vi "Process.vi"(8 "error in":errorcluster, 11 "Instrument.DAQ":refnum<class "Instrument.DAQ.lvclass">) -> (0 "error out":errorcluster, 3 "Instrument.DAQ out":refnum<class "Instrument.DAQ.lvclass">)   [LabVIEW 2019, in "Instrument.Lockin.lvlib" / "Instrument.DAQ.lvclass"]
doc: "---------------------------------------------------------------\nJKI State Machine Objects™\nhttp://jki.net/state-machine-objects/\nCopyright (C) 2005-2015, JKI <info@jki.net>\nALL RIGHTS RESERVED"
uses:
  Instrument.DAQ.lvclass
  C:/Program Files/National Instruments/LabVIEW 2019/vi.lib/JKI/JKI SMO/SMO/SMO.lvclass
  Typedefs/Status--enum.ctl
  Typedefs/DAQ.Config.AO.Range--enum.ctl
  Typedefs/DAQ.Type--enum.ctl
  Typedefs/DAQ.Config.AI.Coupling--enum.ctl
  Typedefs/DAQ.Config.AI.Range--enum.ctl
  DAQmx/typedefs/DAQmx.Status--enum.ctl
  Instrument.DAQ.lvclass/Instrument.DAQ.ctl
  Typedefs/Channel.Gain--Cluster.ctl
  Generator/typedefs/Generator.Sweep Status--enum.ctl
  Typedefs/PublicEvents--DAQ.getSweepWaveforms.ctl
  Typedefs/Results--Cluster.ctl
  <vilib>/JKI/JKI SMO/SMO/SMO.lvclass/SMO.ctl
  Typedefs/PrivateEvents--DAQ.setCalibration.ctl
  support/Simulate/Waveguide Model--Cluster.ctl
  Typedefs/PublicEvents--DAQ.getWaveforms.ctl
  Generator/typedefs/Generator.Command--enum.ctl
  6518129d-eb05-4862-8e0f-948d46b99fe2.vi
  19e91f76-1afa-420f-8f76-37c2ee2699b4.vi
  <vilib>/JKI/JKI SMO/SMO/Private/ReftoDVR--SMO.vi
  <vilib>/dlg_ctls.llb/Space Constant.vi
  <vilib>/AdvancedString/1D String Array to Delimited String.vi
  <vilib>/measure/madcrms.llb/Basic Averaged DC-RMS for N Chan.vi
  <vilib>/JKI/JKI SMO/SMO/SMO.lvclass
  <vilib>/measure/NI_MAPro.lvlib
  Instrument.Lockin/Instrument.Lockin.lvclass
  <userlib>/LevyLab/Debug/Debug.lvlib
  DAQmx/DAQmx.lvclass
  DSP/DSP.lvclass
  Waveform.Attributes/Waveform.Attributes.lvlib
  Generator/Generator.lvclass
panel:
  in  "Tab Control":enum32{"Default", "Advanced"}(tab)
  out "Sweep Chart":dbl(graph)
  out "Generator Chart":u32(graph)
  out "DSP Chart":dbl(graph)
  out "Total Chart":dbl(graph)
  out "sweep status":string
  out "Sweep Start":dbl format="%<%.3X>T"
  out "Status":T1=enum."created"
  in  "Calibrate Phase":bool
  in  "Reset Phase":bool
  out "Total (s)":dbl format="%06_6p"
  in  "Auto Phase":bool
  in  "Zero Offset":bool
  in  "Measure Offset":bool
  out "s.h.":string caption="State History"
  out "Payload":variant
  out "Generate (ms)":u32
  out "DSP (s)":dbl format="%0#6_6p"
  in  "Reset REF":bool
  out "Method":string
  out "DAQmx Status":T2
  out "start sweep":string
  out "reset":string
  in  "DAQ AO":T5(array[cluster]) {"configuration" items=["Default"=-1, "Differential"=10106, "Pseudodifferential"=12529]}
  in  "DAQ AI":T8(array[cluster]) {"configuration" items=["default"=-1, "Differential"=10106, "Pseudodifferential"=12529]; "Coupling" items=[""=0, "AC"=10045, "DC"=10050, "GND"=10066]}
  # "For instructions on how to use the JKI State Machine Objects, examples and video tutorials, visit:\nhttp://jki.net/state-machine-objects/\n\nJKI State Machine Objects™\nhttp://jki.net/state-machine-objects/\nCopyright (C) 2005-2015, JKI <info@jki.net>\nALL RIGHTS RESERVED"
  # "DAQ"
  # "State"
  # "Messages"
  # "Sweep"
  # "Controls"
  # "Timing"
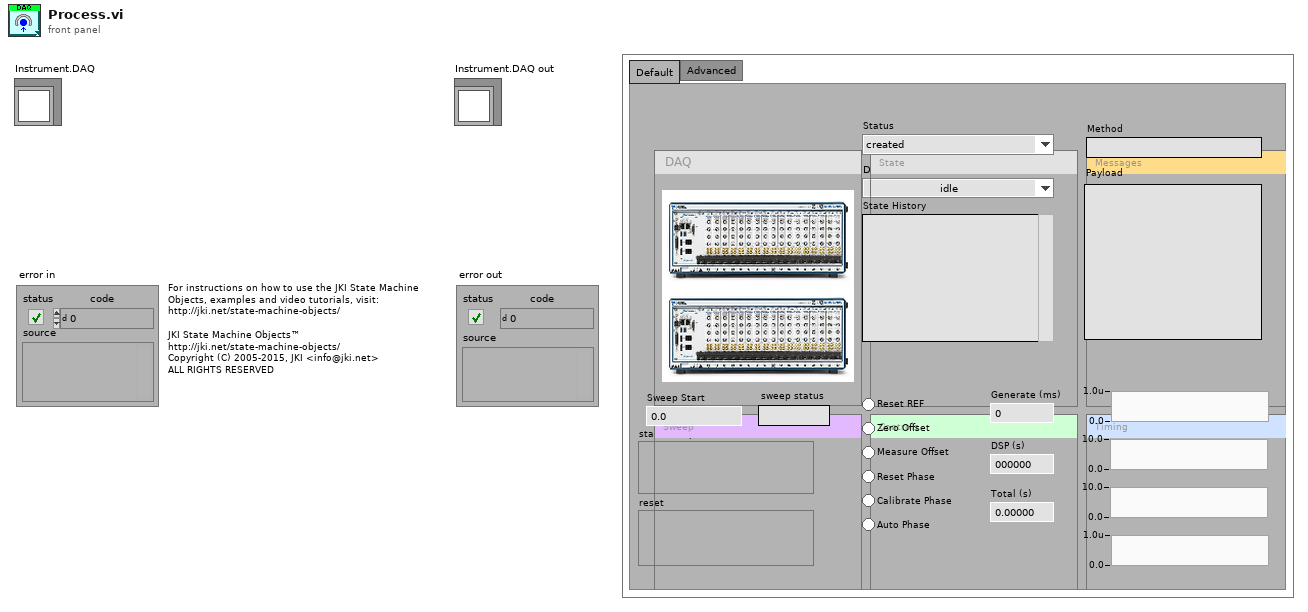
[diagram p1: front panel]
types:
  T1 = typedef "Instrument.Lockin.lvlib/Instrument.DAQ.lvclass/Status--enum.ctl" = enum16{"idle", "created", "started", "stopped", "sweeping"}
  T2 = typedef "DAQmx.lvclass/DAQmx.Status--enum.ctl" = enum16{"idle", "calibrating", "configuring", "creating", "created", "starting", "started", "stopping", "stopped", "clearing", "error"}
  T3 = typedef "Instrument.Lockin.lvlib/Instrument.DAQ.lvclass/DAQ.Config.AO.Range--enum.ctl" = enum16{"±0.1", "±1.0", "±3.5", "±10.0", ""}
  T4 = typedef "Instrument.Lockin.lvlib/Instrument.DAQ.lvclass/DAQ.Type--enum.ctl" = enum16{"None", "USB-4431", "PXI-446x"}
  T5 = cluster{"Channel":tag, "Range":T3, "configuration":i32, "Type":T4}[]
  T6 = typedef "Instrument.Lockin.lvlib/Instrument.DAQ.lvclass/DAQ.Config.AI.Coupling--enum.ctl" = u16
  T7 = typedef "Instrument.Lockin.lvlib/Instrument.DAQ.lvclass/DAQ.Config.AI.Range--enum.ctl" = enum16{"±0.316", "±1.00", "±3.16", "±10.0", "±31.6", "±42.4", ""}
  T8 = cluster{"Channel":tag, "Coupling":T6, "Range":T7, "configuration":i32, "Type":T4}[]
  T9 = typedef "Instrument.Lockin.lvlib/Instrument.DAQ.lvclass/Channel.Gain--Cluster.ctl" = cluster{"Channel":string, "Gain":dbl}
  T10 = enum32{"invalid app kind", "Development System", "Run Time System", "Student Edition", "Embedded LabVIEW", "Evaluation", "Custom"}
  T11 = typedef "Instrument.Lockin.lvlib/Instrument.DAQ.lvclass/PublicEvents--DAQ.getSweepWaveforms.ctl" = cluster{"AO":waveform(dbl)[], "AI":waveform(dbl)[], "X":waveform(dbl)[], "Y":waveform(dbl)[]}
  T12 = enum32{"Invalid", "Standard", "Closed", "Hidden", "Minimized", "Maximized"}
  T13 = typedef "Generator.lvclass/Generator.Sweep Status--enum.ctl" = enum16{"idle", "initializing", "waiting", "sweeping", "stopping"}
  T14 = typedef "Instrument.Lockin.lvlib/Instrument.DAQ.lvclass/PrivateEvents--DAQ.setCalibration.ctl" = enum16{"Check", "Calibrate"}
  T15 = typedef "Instrument.Lockin.lvlib/Instrument.DAQ.lvclass/Waveguide Model--Cluster.ctl" = cluster{"I+":i32, "I-":i32, "V+":i32, "V-":i32, "Vsg":i32}
  T16 = typedef "Instrument.Lockin.lvlib/Instrument.DAQ.lvclass/PublicEvents--DAQ.getWaveforms.ctl" = cluster{"AO":waveform(dbl)[], "AI":waveform(dbl)[], "REF_X":waveform(dbl)[], "REF_Y":waveform(dbl)[], "X":waveform(dbl)[], "Y":waveform(dbl)[]}
  T17 = typedef "Generator.lvclass/Generator.Command--enum.ctl" = enum16{"start", "stop", "start sweep", "stop sweep"}
  T18 = typedef "Instrument.Lockin.lvlib/Instrument.DAQ.lvclass/Results--Cluster.ctl" = cluster{"Time Stamp":timestamp, "Results (Dictionary)":cluster{"key":string, "value":dbl[]}[]}
  T19 = cluster{"Core":cluster{"Current VI Reference":refnum<vi>, "Close Panel on Exit?":bool, "Last Error":cluster{"error":errorcluster, "previous state":string, "remaining states":string}, "Shutdown?":bool}, "SMO":refnum<class "Instrument.DAQ.lvclass">, "DAQ Status":T1, "DAQmx Status":T2, "Sweep Status":T13, "Results":T18, "SweepWaveforms":T11, "Measure Offset":bool, "Saved Amplitudes":dbl[]}
  T20 = typedef "Instrument.Lockin.lvlib/Instrument.DAQ.lvclass/DAQ.Config.AO--Cluster--Array.ctl" = cluster{"Channels":tag, "Range":T3, "terminal configuration":T21, "Type":T4}[]
  T21 = typedef "Instrument.Lockin.lvlib/Instrument.DAQ.lvclass/DAQ.TerminalConfiguration--ring.ctl" = i32
  T22 = cluster{"Channels":tag, "Range":T3, "terminal configuration":T21, "Type":T4}
  T23 = typedef "Instrument.Lockin.lvlib/Instrument.DAQ.lvclass/DAQ.Config.AI--Cluster--Array.ctl" = cluster{"Channels":tag, "Coupling":T6, "Range":T7, "terminal configuration":T21, "Type":T4}[]
  T24 = typedef "Instrument.Lockin.lvlib/Instrument.DAQ.lvclass/Simulation Mode--enum.ctl" = enum16{"AI = HW simulated", "AI = noise*AO", "AI = waveguide"}
  T25 = cluster{"AI Configuration":T23, "Simulation mode":T24}
  T26 = cluster{"Channels":tag, "Coupling":T6, "Range":T7, "terminal configuration":T21, "Type":T4}
  T27 = typedef "Instrument.Lockin.lvlib/Instrument.DAQ.lvclass/AO.Channel--Cluster--Array.ctl" = T28[]
  T28 = typedef "Instrument.Lockin.lvlib/Instrument.DAQ.lvclass/AO.Channel--Cluster.ctl" = cluster{"Enable?":bool, "Channel":i32, "Amplitude":dbl, "Offset":dbl, "Frequency":dbl, "Phase":dbl, "Function":T29, "Sweeping?":bool, "Limit AC":bool, "Limit DC?":bool, "Duty Cycle":bool}
  T29 = typedef "Instrument.Lockin.lvlib/Instrument.DAQ.lvclass/AO.Channel.Function--Enum.ctl" = enum16{"sine", "square", "triangle", "saw"}
  T30 = typedef "Instrument.Lockin.lvlib/Instrument.DAQ.lvclass/AI.Channel--Cluster--Array.ctl" = T31[]
  T31 = typedef "Instrument.Lockin.lvlib/Instrument.DAQ.lvclass/AI.Channel--Cluster.ctl" = cluster{"Enable?":bool, "Channel":i32, "References":u16[], "reference index":i32}
  T32 = typedef "Instrument.Lockin.lvlib/Instrument.DAQ.lvclass/REF.Channel--Cluster--Array.ctl" = T33[]
  T33 = typedef "Instrument.Lockin.lvlib/Instrument.DAQ.lvclass/REF.Channel--Cluster.ctl" = cluster{"Enable?":bool, "Channel":i32, "Frequency":dbl, "Phase":dbl, "TC":dbl, "Roll-Off":i32}
  T34 = typedef "Instrument.Lockin.lvlib/Instrument.DAQ.lvclass/DAQ.Sampling--Cluster.ctl" = cluster{"Sampling":T35, "sample mode":i32, "Fs Mode":T36, "Fs Multiplier":dbl, "Refresh Rate (Hz)":dbl, "Decimation.PreDSP":i32, "Decimation.PostDSP":i32, "Fs.Output":dbl}
  T35 = typedef "Instrument.Lockin.lvlib/Instrument.DAQ.lvclass/DAQ.Sampling.Sampling--Cluster.ctl" = cluster{"Fs":dbl, "#s":i32}
  T36 = typedef "Instrument.Lockin.lvlib/Instrument.DAQ.lvclass/DAQ.Sampling.Fs Mode--enum.ctl" = enum16{"Manual", "Auto Fs", "Max Fs"}
  T37 = typedef "Instrument.Lockin.lvlib/Instrument.DAQ.lvclass/Sweep.Configuration--Cluster.ctl" = cluster{"sweepTime":dbl, "initialWaitTime":dbl, "returnToStart":bool, "sweepChannels":T38}
  T38 = typedef "Instrument.Lockin.lvlib/Instrument.DAQ.lvclass/Sweep.Channel--Cluster--Array.ctl" = T39[]
  T39 = typedef "Instrument.Lockin.lvlib/Instrument.DAQ.lvclass/Sweep.Channel--Cluster.ctl" = cluster{"Enable?":bool, "Channel":u16, "Start":dbl, "End":dbl, "Pattern":T40, "Table":dbl[]}
  T40 = typedef "Instrument.Lockin.lvlib/Instrument.DAQ.lvclass/Sweep.Pattern--Enum.ctl" = enum16{"Ramp /", "Ramp /\\", "Smooth Ramp _/", "Smooth Ramp _/\\_", "Table"}
  T41 = typedef "Instrument.Lockin.lvlib/Instrument.DAQ.lvclass/PrivateEvents--DAQ.measureOffset.ctl" = bool
  T42 = typedef "Instrument.Lockin.lvlib/Instrument.DAQ.lvclass/PrivateEvents--DAQ.zeroPhase.ctl" = bool
  T43 = typedef "Instrument.Lockin.lvlib/Instrument.DAQ.lvclass/Configuration.Prefilter--Cluster.ctl" = cluster{"60 Hz":bool, "Low Pass":bool, "Low Pass Cutoff (Hz)":dbl}
  T44 = typedef "Instrument.Lockin.lvlib/Instrument.DAQ.lvclass/Configuration.AmplitudeLimit--Cluster.ctl" = cluster{"Limit?":bool, "Limit (V)":dbl}
  T45 = typedef "Instrument.Lockin.lvlib/Instrument.DAQ.lvclass/Configuration.DCLimit--Cluster.ctl" = cluster{"Limit?":bool, "Limit (V)":dbl}
  T46 = typedef "Instrument.Lockin.lvlib/Instrument.DAQ.lvclass/Configuration.DutyCycle--Cluster.ctl" = cluster{"Option?":bool, "Duty Cycle (%)":dbl}
  T47 = typedef "Instrument.Lockin.lvlib/Instrument.DAQ.lvclass/Configuration.LinkFrequencies--Cluster.ctl" = cluster{"Link?":bool, "Frequency (Hz)":dbl}
  T48 = typedef "Instrument.Lockin.lvlib/Instrument.DAQ.lvclass/State--enum.ctl" = enum16{"start", "stop", "reset", "start sweep", "stop sweep"}
  T49 = typedef "Instrument.Lockin.lvlib/Instrument.DAQ.lvclass/PrivateEvents--DAQ.showUI.ctl" = bool
  T50 = typedef "DAQmx.lvclass/DeviceInfo--Cluster.ctl" = cluster{"DeviceName":string, "DevIsSimulated":bool, "DeviceSerialNumber":string, "ProductType":string, "ProductCategory":i32, "ProductNumber":u32, "ChassisNumber":u32, "SlotNumber":u32, "ChassisName":string, "ChassisSerialNumber":string, "DevTemp":dbl, "SelfCal.LastDate/Time":string, "SelfCal.LastTemp":dbl, "calibration due?":bool}
  T51 = cluster{"Active Device":string, "SelfCal.LastDate/Time":string, "SelfCal.LastTemp":dbl, "DevTemp":dbl, "calibration due?":bool}[]
  T52 = typedef "Instrument.Lockin.lvlib/Instrument.DAQ.lvclass/DAQ.Calibration--Cluster.ctl" = cluster{"Active Device":string, "SelfCal.LastDate/Time":dbl, "SelfCal.LastTemp":dbl, "DevTemp":dbl, "calibration due?":bool}
  T53 = typedef "eventsource.ctl" = u32
  T54 = typedef "DAQmx.lvclass/DAQ.Config.Timing.Sampling--Cluster.ctl" = cluster{"Fs":dbl, "#s":i32}
  T55 = typedef "DAQmx.lvclass/DAQ.Config.Timing.Fs Mode--enum.ctl" = enum16{"Manual", "Auto Fs", "Max Fs"}
  T56 = typedef "DAQmx.lvclass/DAQ.Config.AO--Cluster--Array.ctl" = T57[]
  T57 = typedef "DAQmx.lvclass/DAQ.Config.AO--Cluster.ctl" = cluster{"Channels":tag, "Range":T58, "output terminal configuration":i32, "Type":T59}
  T58 = typedef "DAQmx.lvclass/DAQ.Config.AO.Range--enum.ctl" = enum16{"±0.1", "±1.0", "±3.5", "±10.0", ""}
  T59 = typedef "DAQmx.lvclass/DAQ.Config.Device Type--enum.ctl" = enum16{"None", "USB-4431", "PXI-446x"}
  T60 = typedef "DAQmx.lvclass/DAQ.Config.AI--Cluster--Array.ctl" = T61[]
  T61 = typedef "DAQmx.lvclass/DAQ.Config.AI--Cluster.ctl" = cluster{"Channels":tag, "Coupling":T62, "Range":T63, "input terminal configuration":i32, "Type":T59}
  T62 = typedef "DAQmx.lvclass/DAQ.Config.AI.Coupling--enum.ctl" = u16
  T63 = typedef "DAQmx.lvclass/DAQ.Config.AI.Range--enum.ctl" = enum16{"±0.316", "±1.00", "±3.16", "±10.0", "±31.6", "±42.4", ""}
  T64 = typedef "Generator.lvclass/AO.Channel--Cluster--Array.ctl" = T65[]
  T65 = typedef "Generator.lvclass/AO.Channel--Cluster.ctl" = cluster{"Enable?":bool, "Channel":i32, "Amplitude":dbl, "Offset":dbl, "Frequency":dbl, "Phase":dbl, "Function":T66, "Sweeping?":bool, "Limit AC?":bool, "Limit DC?":bool, "Duty Cycle?":bool, "Duty Cycle":dbl}
  T66 = typedef "Generator.lvclass/AO.Channel.Function--Enum.ctl" = enum16{"sine", "square", "triangle", "saw"}
  T67 = cluster{"Current VI Reference":refnum<vi>, "Close Panel on Exit?":bool, "Last Error":cluster{"error":errorcluster, "previous state":string, "remaining states":string}, "Shutdown?":bool}
  T68 = typedef "Instrument.Lockin.lvlib/Instrument.DAQ.lvclass/DeviceInfo--Cluster.ctl" = cluster{"DeviceName":string, "DevIsSimulated":bool, "DeviceSerialNumber":string, "ProductType":string, "ProductCategory":i32, "ProductNumber":u32, "ChassisNumber":u32, "SlotNumber":u32, "ChassisName":string, "ChassisSerialNumber":string, "DevTemp":dbl, "SelfCal.LastDate/Time":string, "SelfCal.LastTemp":dbl, "calibration due?":bool}
  T69 = typedef "Instrument.Lockin.lvlib/Instrument.DAQ.lvclass/DAQ.Calibration--Cluster--Array.ctl" = T52[]
  T70 = typedef "Instrument.Lockin.lvlib/Instrument.DAQ.lvclass/DAQ.Configuration--Cluster--Array.ctl" = T71[]
  T71 = typedef "Instrument.Lockin.lvlib/Instrument.DAQ.lvclass/DAQ.Configuration--Cluster.ctl" = cluster{"Device":string, "Lockin.AO":string, "AO.Ch":string, "AO.Range":T3, "AO terminal config":T21, "Lockin.AI":string, "AI.Ch":string, "AI.Range":T7, "AI.Coupling":T6, "AI terminal config":T21}
  T72 = typedef "Instrument.Lockin.lvlib/Instrument.DAQ.lvclass/Channel.Gain--Cluster--Array.ctl" = T9[]
  T73 = typedef "Debug.lvlib/Attribute.Debug.lvclass/DebugBehavior.ctl" = enum16{"Normal", "Debug"}
  T74 = typedef "SMO.lvclass/Protected Events.ctl" = cluster{"StopProcesses":refnum<user-event>, "AbortProcesses":refnum<user-event>, "Config Changed":refnum<user-event>, "Dependency":refnum<user-event>}
  T75 = typedef "Instrument.Lockin.lvlib/Instrument.DAQ.lvclass/PrivateEvents--Cluster.ctl" = cluster{"setAOconfig":refnum<user-event>, "setAIconfig":refnum<user-event>, "setAO":refnum<user-event>, "setREF":refnum<user-event>, "setSampling":refnum<user-event>, "setState":refnum<user-event>, "setInputGain":refnum<user-event>, "setOutputGain":refnum<user-event>, "setSweep":refnum<user-event>, "measureOffset":refnum<user-event>, "zeroOffset":refnum<user-event>, "setPreFilter":refnum<user-event>, "autoConfigureDAQ":refnum<user-event>, "setCalibration":refnum<user-event>, "setAI":refnum<user-event>, "zeroPhase":refnum<user-event>, "setAmplitudeLimit":refnum<user-event>, "setLinkFrequencies":refnum<user-event>, "showUI":refnum<user-event>, "setInputOffset":refnum<user-event>, "setDCLimit":refnum<user-event>, "setDutyCycle":refnum<user-event>}
  T76 = typedef "DAQmx.lvclass/PublicEvents--Cluster.ctl" = cluster{"Status":refnum<user-event>, "Devices":refnum<user-event>, "Calibration":refnum<user-event>, "Timing":refnum<user-event>, "AOconfig":refnum<user-event>, "AIconfig":refnum<user-event>, "Waveforms":refnum<user-event>}
  T77 = typedef "Generator.lvclass/PublicEvents--Cluster.ctl" = cluster{"Status":refnum<user-event>, "SweepStatus":refnum<user-event>, "AOChannels":refnum<user-event>, "Waveforms":refnum<user-event>}
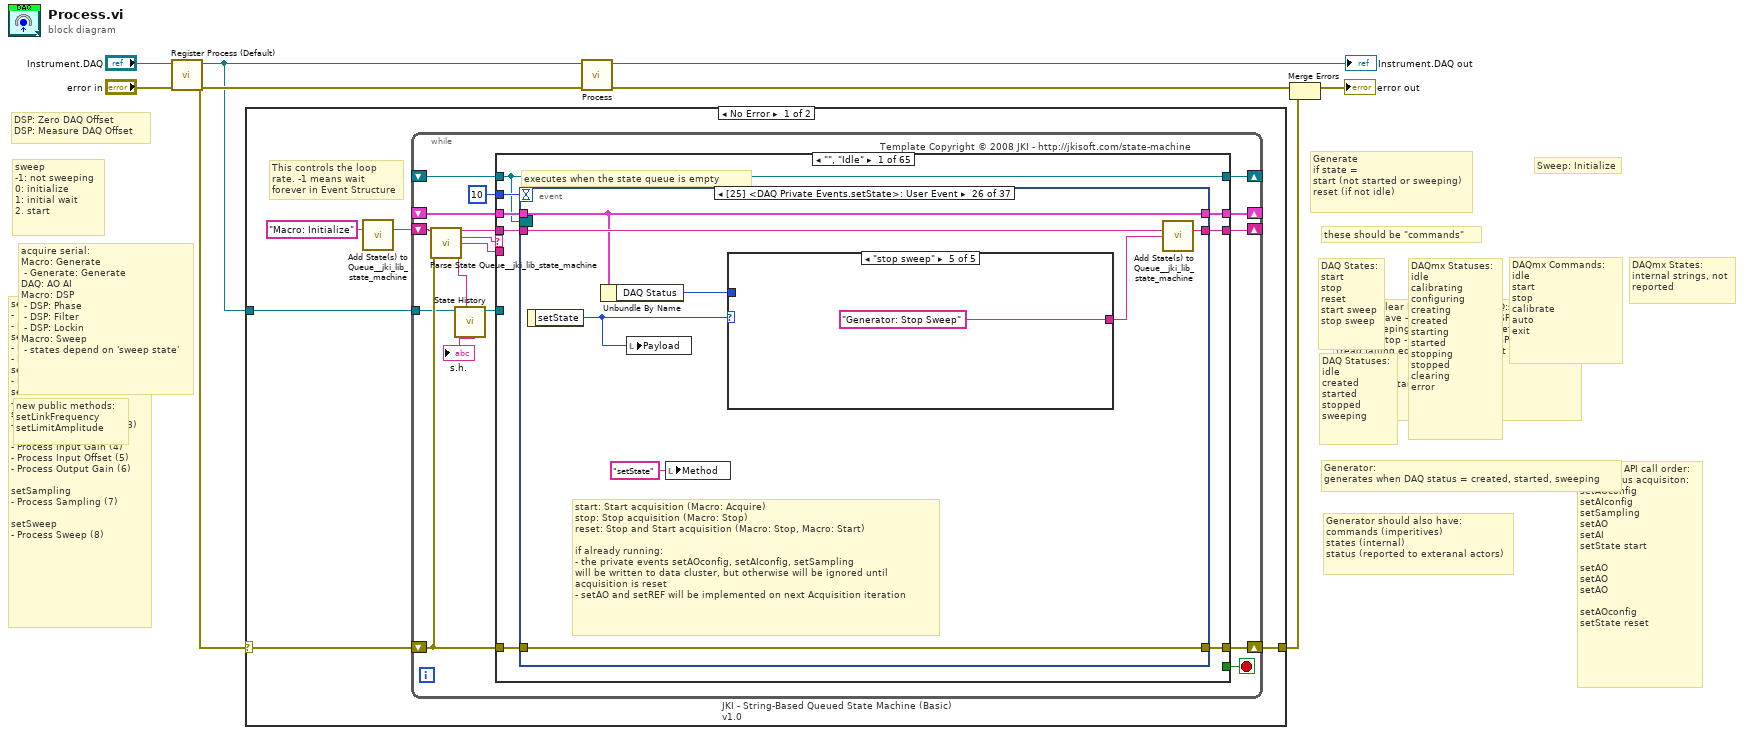
[diagram p0: block diagram]
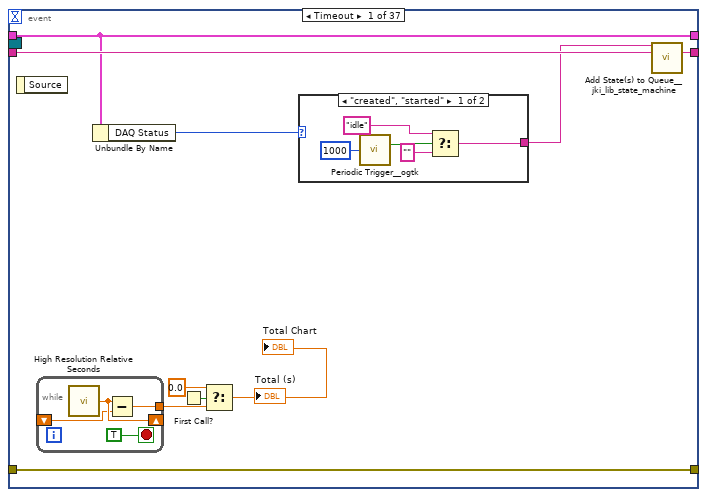
[diagram p2: hidden frame]
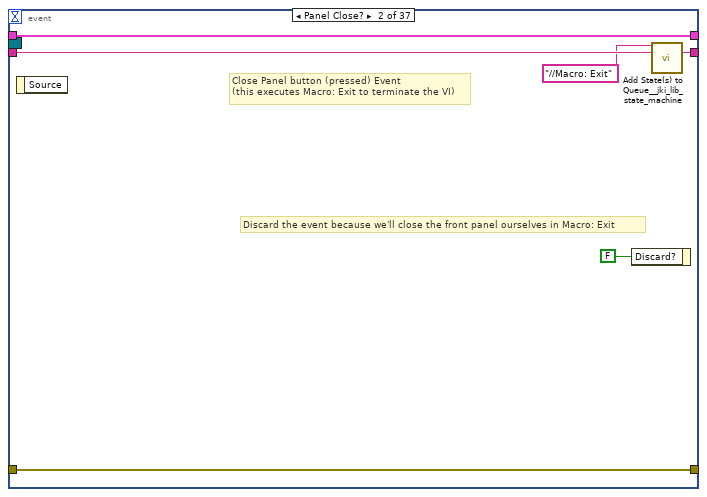
[diagram p4: hidden frame]
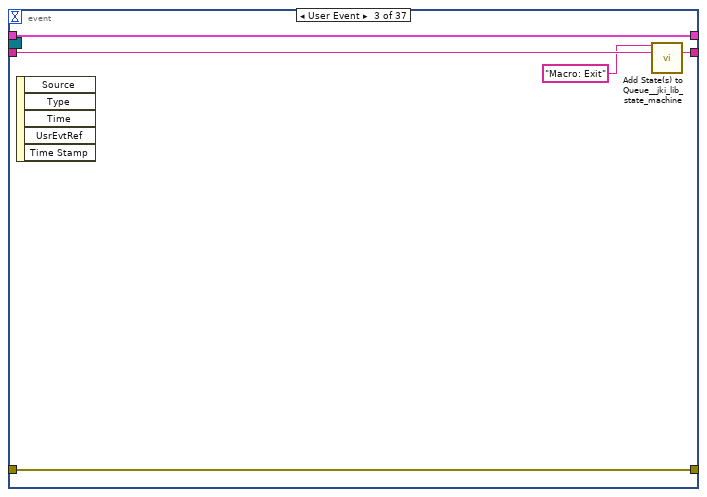
[diagram p5: hidden frame]
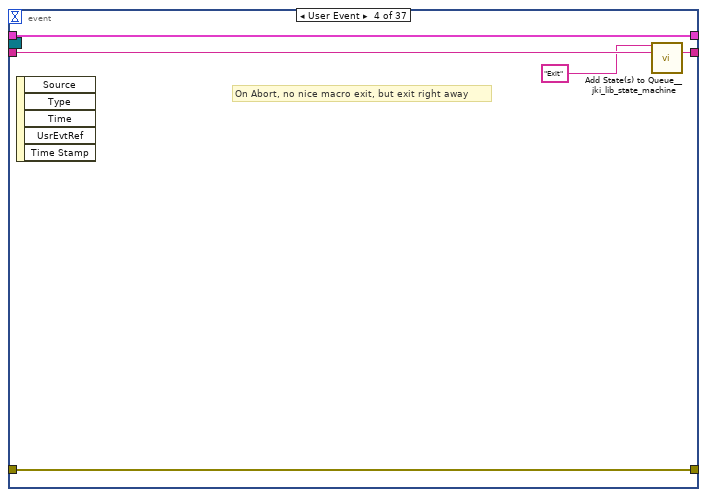
[diagram p6: hidden frame]
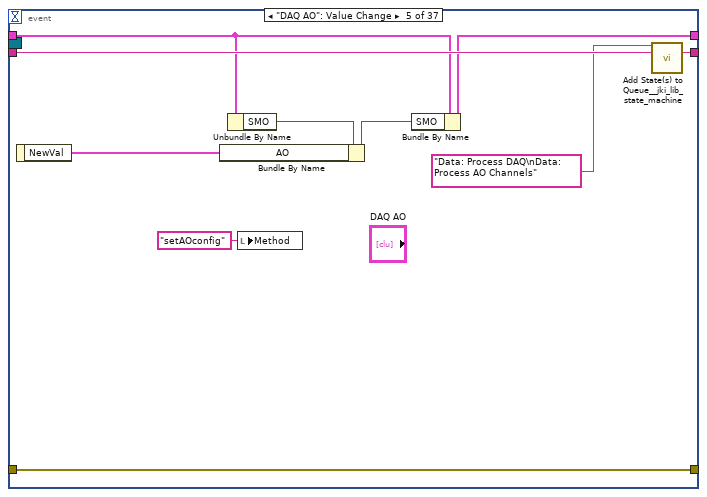
[diagram p7: hidden frame]
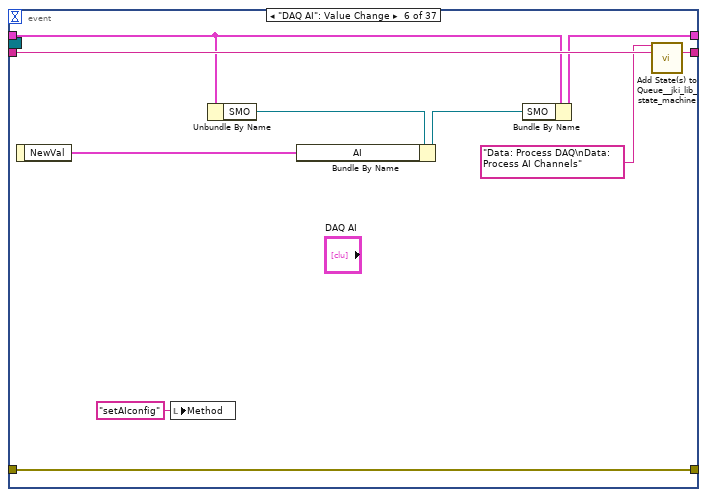
[diagram p8: hidden frame]
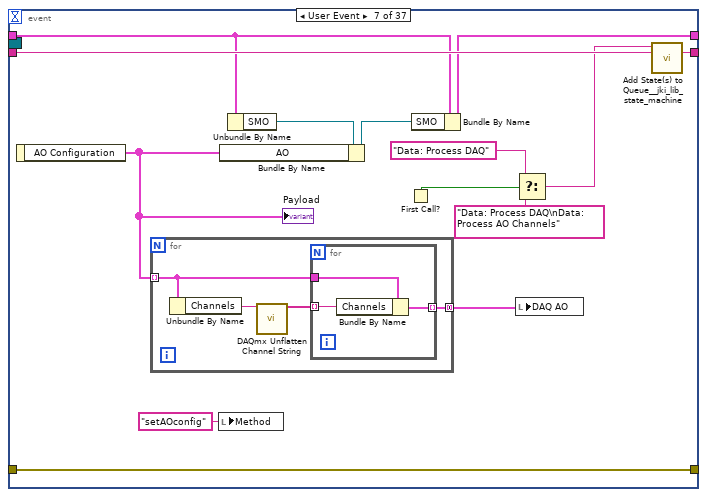
[diagram p9: hidden frame]
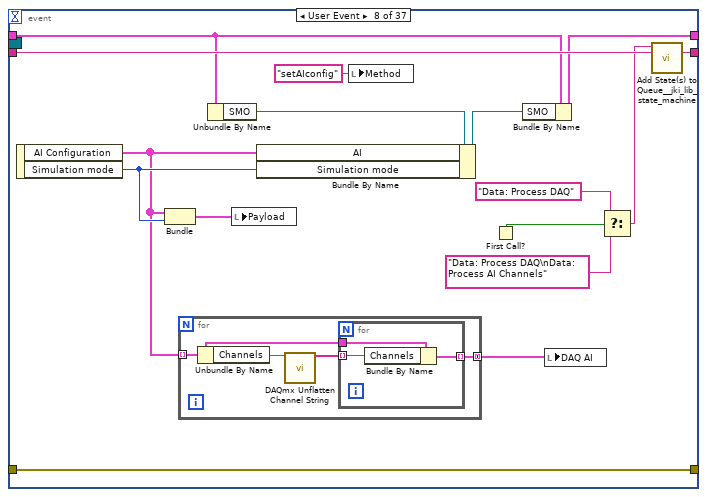
[diagram p10: hidden frame]
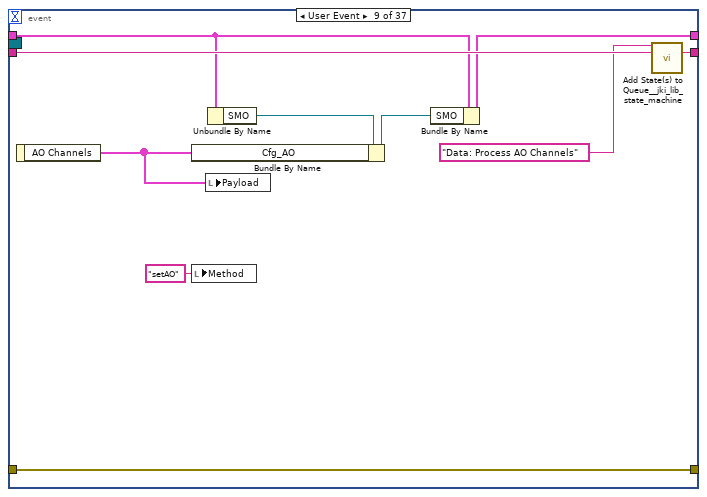
[diagram p11: hidden frame]
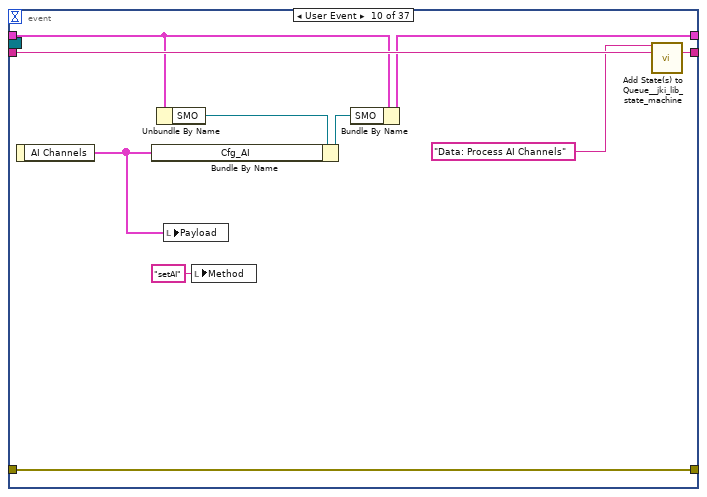
[diagram p12: hidden frame]
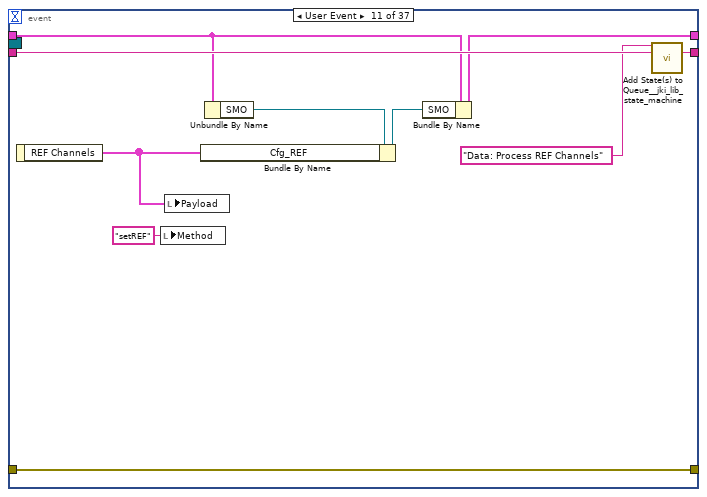
[diagram p13: hidden frame]
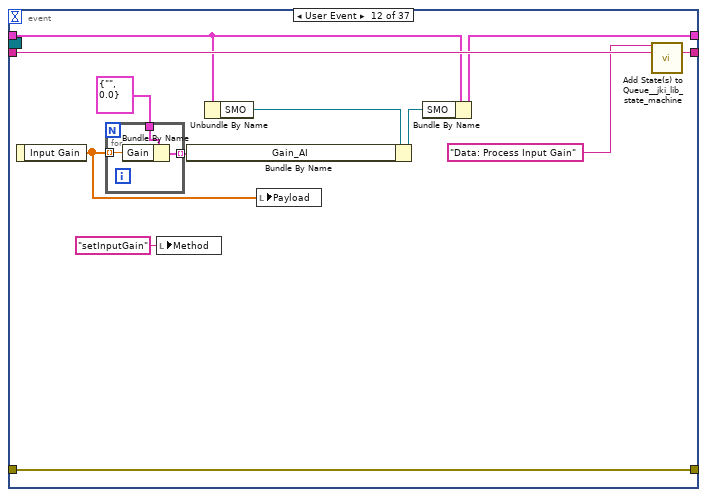
[diagram p14: hidden frame]
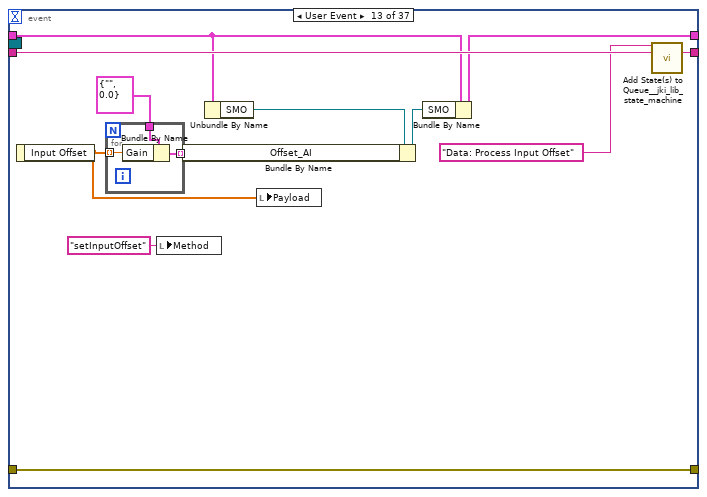
[diagram p15: hidden frame]
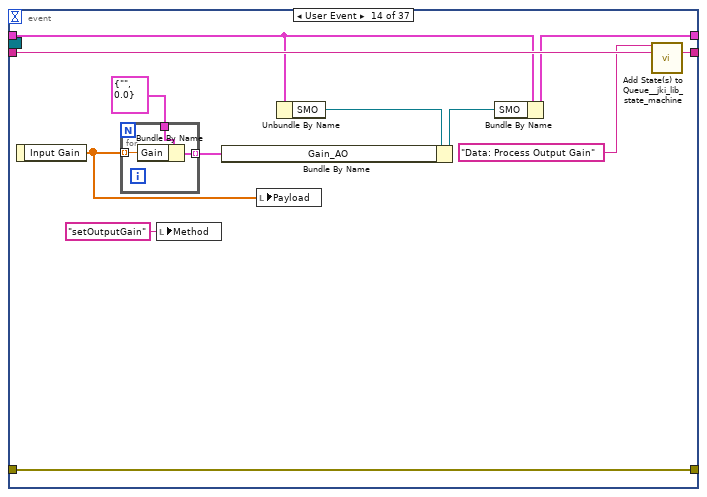
[diagram p16: hidden frame]
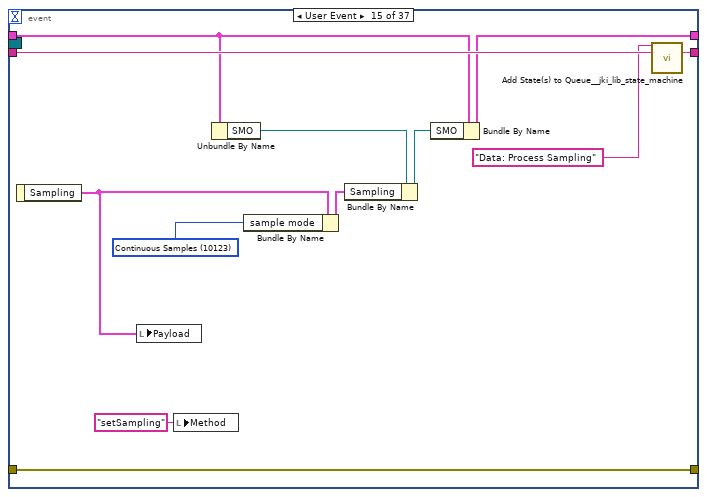
[diagram p17: hidden frame]
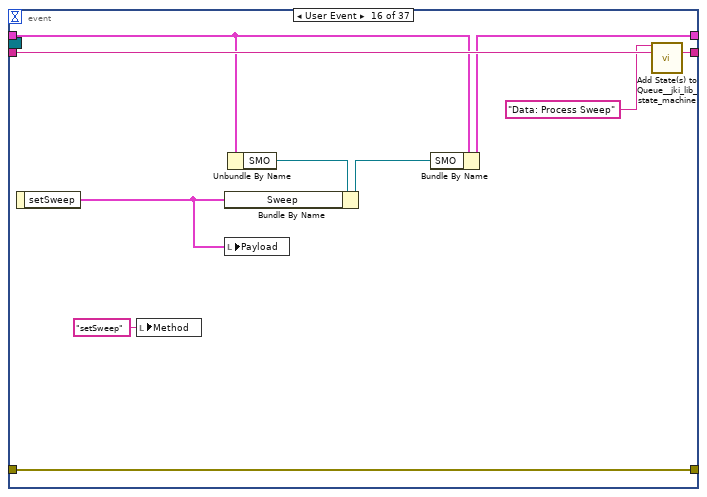
[diagram p18: hidden frame]
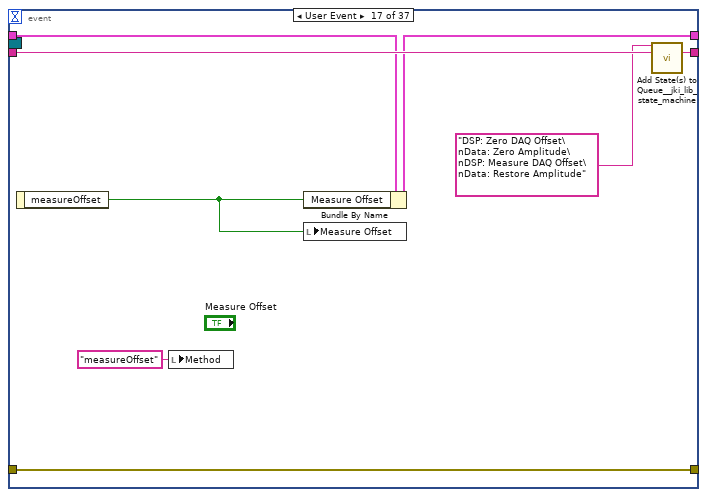
[diagram p19: hidden frame]
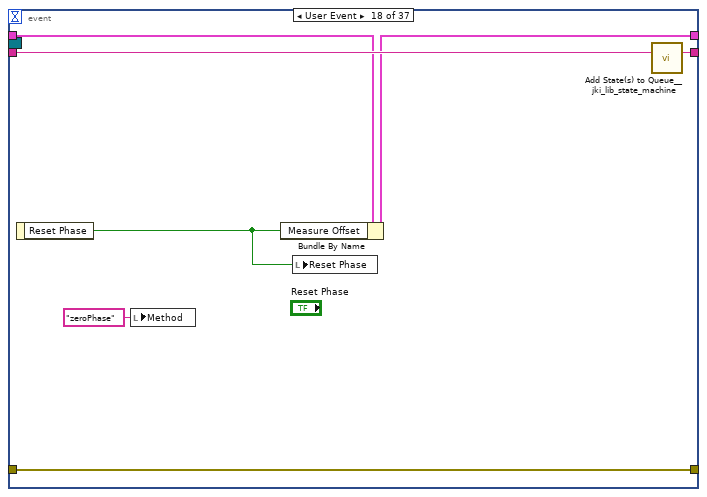
[diagram p20: hidden frame]
diagram:
  # "Sweep: Initialize"
  # "- Sweep: Clear Data - called by DAQ:setState\n- Sweep: Save - called by Macro: DSP\n(read sweeping attribute from waveform)\n- Sweep: Stop - called by Macro: DSP\n(read falling edge sweeping --> not sweeping)\n\n\nGenerator: Start, Stop"
  # "example API call order:\ncontinuous acquisiton:\nsetAOconfig\nsetAIconfig\nsetSampling\nsetAO\nsetAI\nsetState start\n\nsetAO\nsetAO\nsetAO\n\nsetAOconfig\nsetState reset"
  # "Generator should also have:\ncommands (imperitives)\nstates (internal)\nstatus (reported to exteranal actors)"
  # "these should be \"commands\""
  # "DAQmx States:\ninternal strings, not\nreported"
  # "DAQmx Commands:\nidle\nstart\nstop\ncalibrate\nauto\nexit"
  # "Generator:\ngenerates when DAQ status = created, started, sweeping"
  # "DAQmx Statuses:\nidle\ncalibrating\nconfiguring\ncreating\ncreated\nstarting\nstarted\nstopping\nstopped\nclearing\nerror"
  # "DAQ Statuses:\nidle\ncreated\nstarted\nstopped\nsweeping"
  # "DAQ States:\nstart\nstop\nreset\nstart sweep\nstop sweep"
  # "Generate\nif state = \nstart (not started or sweeping)\nreset (if not idle)"
  # "setAOconfig:\n-\t Process DAQ (0)\n- Process AO Channels (1)\nsetAOconfig\n- Process DAQ\n- Process AI Channels (2)\nsetAO\n- Process AO Channels\nsetAI\n- Process AI Channels\nsetREF\n- Process REF Channels (3)\n\n- Process Input Gain (4)\n- Process Input Offset (5)\n- Process Output Gain (6)\n\nsetSampling\n- Process Sampling (7)\n\nsetSweep\n- Process Sweep (8)"
  # "acquire serial:\nMacro: Generate\n - Generate: Generate\nDAQ: AO AI\nMacro: DSP\n - DSP: Phase\n - DSP: Filter\n - DSP: Lockin\nMacro: Sweep\n - states depend on 'sweep state'"
  # "sweep\n-1: not sweeping\n0: initialize\n1: initial wait\n2. start"
  # "DSP: Zero DAQ Offset\nDSP: Measure DAQ Offset"
  # "new public methods:\nsetLinkFrequency\nsetLimitAmplitude"
  n1 = call <vilib>:"Register Process (Default).vi"("error in (no error)"="error in", "SMO"="Instrument.DAQ") -> ("error out"=w5:errorcluster, "SelfRef"=w4:refnum<class "Instrument.DAQ.lvclass">)  [unwired: 8 in]
  n2 = case shown="No Error" w5 {
    selector: w5 -> [w13 w1361]
    tunnel: w4 -> [w9 _]
    tunnel: [w12 w1361] -> w1
    frame No Error {
      # "This controls the loop rate. -1 means wait forever in Event Structure"
      n3 = call <vilib>:"Add State(s) to Queue__jki_lib_state_machine.vi"("State(s) in (\"\")"="Macro: Initialize") -> ("States Out"=w11:string)  [unwired: 14 in]
      n4 = while "JKI - String-Based Queued State Machine (Basic) v1.0" {
        shift-right: [w24] -> _
        shift-left: _ -> [w20]
        shift-right: [w19] -> w12
        shift-left: w13 -> [w23]
        shift-right: [w26] -> _
        shift-left: w11 -> [w27]
        tunnel: w9 -> [w14]
        shift-right: [w22] -> _
        shift-left: _ -> [w21]
        stop <- w25 stop-if-true
        # "Template Copyright © 2008 JKI - http://jkisoft.com/state-machine"
        n5 = call <vilib>:"Parse State Queue__jki_lib_state_machine.vi"("State Queue"=w27, "Error In (no error)"=w23) -> ("Remaining States"=w29:string, "Current State"=w17:string, "Arguments"=w28:string)  [unwired: 11 in]
        n6 = call <userlib>:"State History.vi"("Current State"=w17, "SMO"=w14) -> ("SMO"=w15:refnum<class "Instrument.DAQ.lvclass">, "History"=→"s.h.":string)  [unwired: 8 in]
        n7 = case shown="\"\", \"Idle\"" w17 {
          selector: w17 -> [_ _ w479 _ _ _ _ _ _ _ _ _ _ _ _ _ _ _ _ _ _ _ _ _ _ _ _ _ _ w873 _ _ _ _ _ _ _ _ _ _ _ _ _ _ _ _ _ _ _ _ _ _ _ _ _ _ _ _ _ _ _ _ _ _ _]
          tunnel: w29 -> [w37 w477 w483 w502 w504 w521 w526 w541 w552 w573 w583 w599 w628 w649 w674 w694 w706 w718 w730 w747 w756 w771 w781 w793 w817 w838 w854 w859 w868 w884 w891 w907 w939 w948 w963 w982 w1016 w1023 w1040 w1070 w1075 w1086 w1091 w1111 w1117 w1122 w1131 w1140 w1153 w1170 w1175 w1185 w1205 w1235 w1252 w1270 w1290 w1307 w1312 w1319 w1324 w1333 w1342 w1351 w1360]
          tunnel: w28 -> [_ _ _ _ _ _ _ _ _ _ _ w584 w621 _ _ _ _ _ _ _ _ _ _ _ w795 _ _ _ _ w869 w885 w901 _ _ _ _ _ _ _ _ _ _ _ _ _ _ _ _ w1142 _ _ _ _ _ _ _ _ _ _ _ _ _ _ _ _]
          tunnel: w20 -> [w35 w474 w481 w493 w513 w517 w523 _ w546 w568 w574 w595 w624 w645 w670 w690 w701 w714 w725 w743 w752 w765 w777 w789 w813 w832 w848 w856 w866 w881 w889 w903 w936 w944 w951 w971 w1000 w1018 w1034 w1060 w1072 w1083 w1088 w1109 w1115 w1120 w1126 w1137 w1150 w1167 w1173 w1178 w1201 w1232 w1249 w1266 w1287 w1303 w1310 w1313 w1322 w1330 w1339 w1348 w1357]
          tunnel: w23 -> [w33 w475 w484 w499 w505 _ w524 w534 w547 w565 w576 w588 w614 w642 w668 w689 w697 w708 w720 w741 w748 w763 w775 w787 w804 w834 w851 w857 w862 w882 w887 w905 w937 w946 w949 w980 w1014 w1021 w1039 w1055 w1073 w1078 w1089 w1094 w1114 w1118 w1127 w1132 w1147 w1163 w1171 w1180 w1198 w1229 w1238 w1267 w1272 w1300 w1308 w1316 w1320 w1326 w1335 w1344 w1353]
          tunnel: [w36 w476 w482 w501 w508 w520 w525 w540 w551 w572 w582 w598 w627 w648 w673 w693 w705 w717 w729 w746 w755 w770 w780 w792 w816 w837 w853 w858 w867 w883 w890 w906 w938 w947 w962 w981 w1015 w1022 w1037 w1069 w1074 w1085 w1090 w1110 w1116 w1121 w1130 w1139 w1152 w1169 w1174 w1184 w1204 w1234 w1251 w1269 w1289 w1306 w1311 w1318 w1323 w1332 w1341 w1350 w1359] -> w26
          tunnel: [_ _ _ _ _ TRUE _ _ _ _ _ _ _ _ _ _ _ _ _ _ _ _ _ _ _ _ _ _ _ _ _ _ _ _ _ _ _ _ _ _ _ _ _ _ _ _ _ _ _ _ _ _ _ _ _ _ _ _ _ _ _ _ _ _ _] -> w25
          tunnel: [w32 w474 w481 w500 w512 w517 w523 w538 w548 w569 w575 w596 w625 w646 w671 w691 w702 w715 w726 w744 w752 w766 w778 w790 w814 w833 w848 w856 w866 w881 w889 w903 w936 w944 w953 w972 w1001 w1018 w1034 w1060 w1072 w1083 w1088 w1109 w1115 w1120 w1125 w1136 w1149 w1166 w1173 w1179 w1200 w1231 w1248 w1266 w1286 w1302 w1310 w1313 w1322 w1330 w1339 w1348 w1357] -> w24
          tunnel: 10 ("to") -> [w31 _ _ _ _ _ _ _ _ _ _ _ _ _ _ _ _ _ _ _ _ _ _ _ _ _ _ _ _ _ _ _ _ _ _ _ _ _ _ _ _ _ _ _ _ _ _ _ _ _ _ _ _ _ _ _ _ _ _ _ _ _ _ _ _]
          tunnel: w15 -> [_ _ _ _ _ _ _ w533 _ _ _ _ _ _ _ _ _ _ _ _ _ _ _ _ _ _ _ _ _ _ _ _ _ _ _ _ _ _ _ _ _ _ _ _ _ _ _ _ _ _ _ _ _ _ _ _ _ _ _ _ _ _ _ _ _]
          tunnel: [w30 w473 w478 w490 w515 w518 w522 w539 w550 w571 w581 w597 w626 w647 w672 w692 w704 w716 w728 w745 w754 w769 w779 w791 w815 w836 w849 w855 w865 w880 w888 w900 w935 w945 w961 w979 w1009 w1020 w1038 w1068 w1071 w1084 w1087 w1103 w1112 w1119 w1129 w1138 w1151 w1168 w1172 w1183 w1203 w1233 w1250 w1268 w1288 w1305 w1309 w1317 w1321 w1331 w1340 w1349 w1358] -> w22
          tunnel: w21 -> [w30 w473 w478 w490 w515 w518 w522 w539 w550 w571 w581 w597 w626 w647 w672 w692 w704 w716 w728 w745 w754 w769 w779 w791 w815 w836 w849 w855 w865 w880 w888 w900 w935 w945 w961 w979 w1009 w1020 w1038 w1068 w1071 w1084 w1087 _ w1112 w1119 w1129 w1138 w1151 w1168 w1172 w1183 w1203 w1233 w1250 w1268 w1288 w1305 w1309 w1317 w1321 w1331 w1340 w1349 w1358]
          tunnel: [w34 w475 w485 w499 errorcluster {"status"=FALSE, "code"=0, "source"=""} ("No error") w516 w524 w536 w543 w566 w577 w585 w610 w637 w661 w675 w696 w712 w721 w740 w749 w764 w774 w785 w803 w835 w850 w857 w863 w882 w886 w904 w937 w946 w950 w980 w1014 w1021 w1039 w1056 w1073 w1077 w1089 w1107 w1114 w1118 w1123 w1133 w1146 w1162 w1171 w1181 w1191 w1219 w1243 w1267 w1273 w1294 w1308 w1316 w1320 w1327 w1336 w1345 w1354] -> w19
          frame "", "Idle" {
            # "executes when the state queue is empty"
            n8 = event shown="[25] <DAQ Private Events.setState>: User Event" {
              selector: w30 -> [_ _ _ _ _ _ _ _ _ _ _ _ _ _ _ _ _ _ _ _ _ _ _ _ _ _ _ _ _ _ _ _ _ _ _ _ _]
              dyn-events: _ -> [_ _ _ _ _ _ _ _ _ _ _ _ _ _ _ _ _ _ _ _ _ _ _ _ _ _ _ _ _ _ _ _ _ _ _ _ _]
              timeout: w31 -> [_ _ _ _ _ _ _ _ _ _ _ _ _ _ _ _ _ _ _ _ _ _ _ _ _ _ _ _ _ _ _ _ _ _ _ _ _]
              tunnel: w37 -> [w42 w63 w68 w73 w83 w93 w107 w130 w147 w157 w167 w179 w194 w209 w224 w234 w242 w249 w255 w265 w275 w285 w295 w305 w312 w320 w342 w353 w360 w370 w381 w398 w408 w418 w436 w451 w465]
              tunnel: [w47 w62 w67 w72 w82 w92 w106 w129 w146 w156 w166 w178 w193 w208 w223 w233 w241 w248 w254 w264 w274 w284 w294 w304 w311 w319 w341 w352 w361 w371 w382 w399 w409 w419 w437 w450 w466] -> w36
              tunnel: w35 -> [w41 w60 w65 w70 w79 w89 w103 w126 w143 w153 w163 w175 w190 w205 w221 w230 w238 w246 w252 w260 w270 w280 w290 w300 w309 w314 w337 w349 w358 w366 w377 w393 w401 w412 w432 w446 w468]
              tunnel: [w46 w61 w66 w71 w76 w86 w100 w121 w142 w148 w159 w172 w187 w204 w219 w231 w240 w247 w253 w263 w273 w283 w293 w303 w310 w318 w340 w351 w357 w365 w376 w397 w407 w417 w428 w445 w460] -> w34
              tunnel: w33 -> [w46 w61 w66 w71 w76 w86 w100 w121 w142 w148 w159 w172 w187 w204 w219 w231 w240 w247 w253 w263 w273 w283 w293 w303 w310 w318 w340 w351 w357 w365 w376 w397 w407 w417 w427 w444 w467]
              tunnel: [w41 w60 w65 w70 w81 w91 w105 w128 w145 w155 w165 w177 w192 w207 w217 w232 w237 w245 w252 w261 w271 w281 w291 w301 w309 w314 w337 w349 w356 w367 w378 w392 w402 w413 w433 w446 w469] -> w32
              event Timeout {
                n9 = event-data() -> ()  [unwired: 1 in, 1 out]
                n10 = while {
                  shift-right: [w57] -> _
                  shift-left: _ -> [w56]
                  tunnel: [w55] -> w44
                  stop <- TRUE stop-if-true
                  n11 = call <vilib>:"High Resolution Relative Seconds.vi"() -> ("relative seconds"=w57:dbl)
                  n12 = Subtract(x=w57, y=w56) -> (x-y=w55:dbl)
                }
                n13 = Unbundle By Name(w41) -> ("DAQ Status"=w40:T1)
                n14 = First Call?() -> (First Call?: T/F=w43:bool)
                n15 = Select(t=0.0, s=w43, f=w44) -> (s? t:f=→"Total (s)" →"Total Chart":dbl)
                n16 = case shown="\"created\", \"started\"" w40 {
                  tunnel: [w50 "" ("State(s) in Front (\"\")")] -> w39
                  frame "created", "started" {
                    n17 = call <userlib>:"Periodic Trigger__ogtk.vi"("time (ms)"=u32 1000) -> ("Triggered"=w52:bool)  [unwired: 12 in, 2 out]
                    n18 = Select(t="idle" ("State(s) in Front (\"\")"), s=w52, f="") -> (s? t:f=w50:string)
                  }
                  frame "idle", "stopped", "sweeping" {
                  }
                }
                n19 = call <vilib>:"Add State(s) to Queue__jki_lib_state_machine.vi"("State(s) in Front (\"\")"=w39, "State(s) in (\"\")"=w42) -> ("States Out"=w47:string)  [unwired: 13 in]
              }
              event Panel Close? {
                # "Discard the event because we'll close the front panel ourselves in Macro: Exit"
                # "Close Panel button (pressed) Event\n(this executes Macro: Exit to terminate the VI)"
                n20 = event-data() -> ()  [unwired: 1 in, 1 out]
                n21 = event-data("Discard?"=FALSE) -> ()  [unwired: 1 in, 1 out]
                n22 = call <vilib>:"Add State(s) to Queue__jki_lib_state_machine.vi"("State(s) in Front (\"\")"="//Macro: Exit", "State(s) in (\"\")"=w63) -> ("States Out"=w62:string)  [unwired: 13 in]
              }
              event User Event {
                n23 = event-data() -> ()  [unwired: 1 in, 5 out]
                n24 = call <vilib>:"Add State(s) to Queue__jki_lib_state_machine.vi"("State(s) in Front (\"\")"="Macro: Exit", "State(s) in (\"\")"=w68) -> ("States Out"=w67:string)  [unwired: 13 in]
              }
              event User Event {
                # "On Abort, no nice macro exit, but exit right away"
                n25 = event-data() -> ()  [unwired: 1 in, 5 out]
                n26 = call <vilib>:"Add State(s) to Queue__jki_lib_state_machine.vi"("State(s) in Front (\"\")"="Exit", "State(s) in (\"\")"=w73) -> ("States Out"=w72:string)  [unwired: 13 in]
              }
              event "DAQ AO": Value Change {
                n27 = event-data() -> ("NewVal"=w74:T5)  [unwired: 1 in]
                n28 = Unbundle By Name(w79) -> ("SMO"=w78:refnum<class "Instrument.DAQ.lvclass">)
                n29 = Bundle By Name(cluster=w78, "AO"=w74) -> (w77:refnum<class "Instrument.DAQ.lvclass">)
                n30 = local write "Method"("setAOconfig" ("String")) -> ()
                n31 = Bundle By Name(cluster=w79, "SMO"=w77) -> (w81:T19)
                n32 = call <vilib>:"Add State(s) to Queue__jki_lib_state_machine.vi"("State(s) in Front (\"\")"="Data: Process DAQ\nData: Process AO Channels" ("State(s) in Front (\"\")"), "State(s) in (\"\")"=w83) -> ("States Out"=w82:string)  [unwired: 13 in]
              }
              event "DAQ AI": Value Change {
                n33 = event-data() -> ("NewVal"=w84:T8)  [unwired: 1 in]
                n34 = local write "Method"("setAIconfig" ("String")) -> ()
                n35 = Unbundle By Name(w89) -> ("SMO"=w87:refnum<class "Instrument.DAQ.lvclass">)
                n36 = Bundle By Name(cluster=w87, "AI"=w84) -> (w88:refnum<class "Instrument.DAQ.lvclass">)
                n37 = Bundle By Name(cluster=w89, "SMO"=w88) -> (w91:T19)
                n38 = call <vilib>:"Add State(s) to Queue__jki_lib_state_machine.vi"("State(s) in Front (\"\")"="Data: Process DAQ\nData: Process AI Channels" ("State(s) in Front (\"\")"), "State(s) in (\"\")"=w93) -> ("States Out"=w92:string)  [unwired: 13 in]
              }
              event User Event {
                n39 = event-data() -> ("AO Configuration"=w99:T20)  [unwired: 1 in]
                "Payload" <- w99
                n40 = for {
                  tunnel: w99 -> [w108] mode=indexing
                  tunnel: [w109] -> w98 mode=concatenating
                  n41 = Unbundle By Name(w108) -> ("Channels"=w111:tag)
                  n42 = call <vilib>:"DAQmx Unflatten Channel String.vi"("names in"=w111) -> ("names out"=w110:string[])  [unwired: 13 in, 1 out]
                  n43 = for {
                    tunnel: w108 -> [w114]
                    tunnel: w110 -> [w113] mode=indexing
                    tunnel: [w112] -> w109 mode=indexing
                    n44 = Bundle By Name(cluster=w114, "Channels"=w113) -> (w112:T22)
                  }
                }
                n45 = local write "Method"("setAOconfig" ("String")) -> ()
                n46 = Unbundle By Name(w103) -> ("SMO"=w102:refnum<class "Instrument.DAQ.lvclass">)
                n47 = Bundle By Name(cluster=w102, "AO"=w99) -> (w101:refnum<class "Instrument.DAQ.lvclass">)
                n48 = First Call?() -> (First Call?: T/F=w97:bool)
                n49 = Bundle By Name(cluster=w103, "SMO"=w101) -> (w105:T19)
                n50 = local write "DAQ AO"(w98) -> ()
                n51 = Select(t="Data: Process DAQ" ("State(s) in Front (\"\")"), s=w97, f="Data: Process DAQ\nData: Process AO Channels" ("State(s) in Front (\"\")")) -> (s? t:f=w94:string)
                n52 = call <vilib>:"Add State(s) to Queue__jki_lib_state_machine.vi"("State(s) in Front (\"\")"=w94, "State(s) in (\"\")"=w107) -> ("States Out"=w106:string)  [unwired: 13 in]
              }
              event User Event {
                n53 = event-data() -> ("AI Configuration"=w120:T23, "Simulation mode"=w124:T24)  [unwired: 1 in]
                n54 = Bundle("AI Configuration"=w120, "Simulation mode"=w124) -> (w123:T25)  [unwired: 1 in]
                n55 = for {
                  tunnel: w120 -> [w133] mode=indexing
                  tunnel: [w131] -> w119 mode=concatenating
                  n56 = Unbundle By Name(w133) -> ("Channels"=w134:tag)
                  n57 = call <vilib>:"DAQmx Unflatten Channel String.vi"("names in"=w134) -> ("names out"=w132:string[])  [unwired: 13 in, 1 out]
                  n58 = for {
                    tunnel: w133 -> [w137]
                    tunnel: w132 -> [w136] mode=indexing
                    tunnel: [w135] -> w131 mode=indexing
                    n59 = Bundle By Name(cluster=w137, "Channels"=w136) -> (w135:T26)
                  }
                }
                n60 = Unbundle By Name(w126) -> ("SMO"=w122:refnum<class "Instrument.DAQ.lvclass">)
                n61 = local write "Payload"(w123) -> ()
                n62 = Bundle By Name(cluster=w122, "AI"=w120, "Simulation mode"=w124) -> (w125:refnum<class "Instrument.DAQ.lvclass">)
                n63 = local write "Method"("setAIconfig" ("String")) -> ()
                n64 = First Call?() -> (First Call?: T/F=w118:bool)
                n65 = Bundle By Name(cluster=w126, "SMO"=w125) -> (w128:T19)
                n66 = local write "DAQ AI"(w119) -> ()
                n67 = Select(t="Data: Process DAQ" ("State(s) in Front (\"\")"), s=w118, f="Data: Process DAQ\nData: Process AI Channels" ("State(s) in Front (\"\")")) -> (s? t:f=w116:string)
                n68 = call <vilib>:"Add State(s) to Queue__jki_lib_state_machine.vi"("State(s) in Front (\"\")"=w116, "State(s) in (\"\")"=w130) -> ("States Out"=w129:string)  [unwired: 13 in]
              }
              event User Event {
                n69 = event-data() -> ("AO Channels"=w139:T27)  [unwired: 1 in]
                n70 = local write "Method"("setAO" ("String")) -> ()
                n71 = local write "Payload"(w139) -> ()
                n72 = Unbundle By Name(w143) -> ("SMO"=w141:refnum<class "Instrument.DAQ.lvclass">)
                n73 = Bundle By Name(cluster=w141, "Cfg_AO"=w139) -> (w138:refnum<class "Instrument.DAQ.lvclass">)
                n74 = Bundle By Name(cluster=w143, "SMO"=w138) -> (w145:T19)
                n75 = call <vilib>:"Add State(s) to Queue__jki_lib_state_machine.vi"("State(s) in Front (\"\")"="Data: Process AO Channels" ("State(s) in Front (\"\")"), "State(s) in (\"\")"=w147) -> ("States Out"=w146:string)  [unwired: 13 in]
              }
              event User Event {
                n76 = event-data() -> ("AI Channels"=w151:T30)  [unwired: 1 in]
                n77 = Unbundle By Name(w153) -> ("SMO"=w152:refnum<class "Instrument.DAQ.lvclass">)
                n78 = Bundle By Name(cluster=w152, "Cfg_AI"=w151) -> (w149:refnum<class "Instrument.DAQ.lvclass">)
                n79 = local write "Payload"(w151) -> ()
                n80 = local write "Method"("setAI" ("String")) -> ()
                n81 = Bundle By Name(cluster=w153, "SMO"=w149) -> (w155:T19)
                n82 = call <vilib>:"Add State(s) to Queue__jki_lib_state_machine.vi"("State(s) in Front (\"\")"="Data: Process AI Channels" ("State(s) in Front (\"\")"), "State(s) in (\"\")"=w157) -> ("States Out"=w156:string)  [unwired: 13 in]
              }
              event User Event {
                n83 = event-data() -> ("REF Channels"=w161:T32)  [unwired: 1 in]
                n84 = local write "Method"("setREF" ("String")) -> ()
                n85 = local write "Payload"(w161) -> ()
                n86 = Unbundle By Name(w163) -> ("SMO"=w162:refnum<class "Instrument.DAQ.lvclass">)
                n87 = Bundle By Name(cluster=w162, "Cfg_REF"=w161) -> (w160:refnum<class "Instrument.DAQ.lvclass">)
                n88 = Bundle By Name(cluster=w163, "SMO"=w160) -> (w165:T19)
                n89 = call <vilib>:"Add State(s) to Queue__jki_lib_state_machine.vi"("State(s) in Front (\"\")"="Data: Process REF Channels" ("State(s) in Front (\"\")"), "State(s) in (\"\")"=w167) -> ("States Out"=w166:string)  [unwired: 13 in]
              }
              event User Event {
                n90 = event-data() -> ("Input Gain"=w169:dbl[])  [unwired: 1 in]
                n91 = for {
                  tunnel: T9 {"Channel"="", "Gain"=0.0} ("System Cluster") -> [w182]
                  tunnel: w169 -> [w181] mode=indexing
                  tunnel: [w180] -> w168 mode=indexing
                  n92 = Bundle By Name(cluster=w182, "Gain"=w181) -> (w180:T9)
                }
                n93 = local write "Method"("setInputGain" ("String")) -> ()
                n94 = Unbundle By Name(w175) -> ("SMO"=w174:refnum<class "Instrument.DAQ.lvclass">)
                n95 = Bundle By Name(cluster=w174, "Gain_AI"=w168) -> (w173:refnum<class "Instrument.DAQ.lvclass">)
                n96 = local write "Payload"(w169) -> ()
                n97 = Bundle By Name(cluster=w175, "SMO"=w173) -> (w177:T19)
                n98 = call <vilib>:"Add State(s) to Queue__jki_lib_state_machine.vi"("State(s) in Front (\"\")"="Data: Process Input Gain" ("State(s) in Front (\"\")"), "State(s) in (\"\")"=w179) -> ("States Out"=w178:string)  [unwired: 13 in]
              }
              event User Event {
                n99 = event-data() -> ("Input Offset"=w184:dbl[])  [unwired: 1 in]
                n100 = for {
                  tunnel: T9 {"Channel"="", "Gain"=0.0} ("System Cluster") -> [w197]
                  tunnel: w184 -> [w196] mode=indexing
                  tunnel: [w195] -> w183 mode=indexing
                  n101 = Bundle By Name(cluster=w197, "Gain"=w196) -> (w195:T9)
                }
                n102 = local write "Method"("setInputOffset" ("String")) -> ()
                n103 = Unbundle By Name(w190) -> ("SMO"=w189:refnum<class "Instrument.DAQ.lvclass">)
                n104 = Bundle By Name(cluster=w189, "Offset_AI"=w183) -> (w188:refnum<class "Instrument.DAQ.lvclass">)
                n105 = local write "Payload"(w184) -> ()
                n106 = Bundle By Name(cluster=w190, "SMO"=w188) -> (w192:T19)
                n107 = call <vilib>:"Add State(s) to Queue__jki_lib_state_machine.vi"("State(s) in Front (\"\")"="Data: Process Input Offset" ("State(s) in Front (\"\")"), "State(s) in (\"\")"=w194) -> ("States Out"=w193:string)  [unwired: 13 in]
              }
              event User Event {
                n108 = event-data() -> ("Input Gain"=w199:dbl[])  [unwired: 1 in]
                n109 = for {
                  tunnel: T9 {"Channel"="", "Gain"=0.0} ("System Cluster") -> [w212]
                  tunnel: w199 -> [w211] mode=indexing
                  tunnel: [w210] -> w198 mode=indexing
                  n110 = Bundle By Name(cluster=w212, "Gain"=w211) -> (w210:T9)
                }
                n111 = local write "Method"("setOutputGain" ("String")) -> ()
                n112 = local write "Payload"(w199) -> ()
                n113 = Unbundle By Name(w205) -> ("SMO"=w203:refnum<class "Instrument.DAQ.lvclass">)
                n114 = Bundle By Name(cluster=w203, "Gain_AO"=w198) -> (w202:refnum<class "Instrument.DAQ.lvclass">)
                n115 = Bundle By Name(cluster=w205, "SMO"=w202) -> (w207:T19)
                n116 = call <vilib>:"Add State(s) to Queue__jki_lib_state_machine.vi"("State(s) in Front (\"\")"="Data: Process Output Gain" ("State(s) in Front (\"\")"), "State(s) in (\"\")"=w209) -> ("States Out"=w208:string)  [unwired: 13 in]
              }
              event User Event {
                w215 = 10123 items=["Finite Samples"=10178, "Continuous Samples"=10123, "Hardware Timed Single Point"=12522] ("sample mode")
                n117 = event-data() -> ("Sampling"=w214:T34)  [unwired: 1 in]
                n118 = local write "Payload"(w214) -> ()
                n119 = local write "Method"("setSampling" ("String")) -> ()
                n120 = Unbundle By Name(w221) -> ("SMO"=w220:refnum<class "Instrument.DAQ.lvclass">)
                n121 = Bundle By Name(cluster=w214, "sample mode"=w215) -> (w213:T34)
                n122 = Bundle By Name(cluster=w220, "Sampling"=w213) -> (w218:refnum<class "Instrument.DAQ.lvclass">)
                n123 = Bundle By Name(cluster=w221, "SMO"=w218) -> (w217:T19)
                n124 = call <vilib>:"Add State(s) to Queue__jki_lib_state_machine.vi"("State(s) in Front (\"\")"="Data: Process Sampling" ("State(s) in Front (\"\")"), "State(s) in (\"\")"=w224) -> ("States Out"=w223:string)  [unwired: 13 in]
              }
              event User Event {
                n125 = event-data() -> ("setSweep"=w226:T37)  [unwired: 1 in]
                n126 = local write "Method"("setSweep" ("String")) -> ()
                n127 = local write "Payload"(w226) -> ()
                n128 = Unbundle By Name(w230) -> ("SMO"=w229:refnum<class "Instrument.DAQ.lvclass">)
                n129 = Bundle By Name(cluster=w229, "Sweep"=w226) -> (w228:refnum<class "Instrument.DAQ.lvclass">)
                n130 = Bundle By Name(cluster=w230, "SMO"=w228) -> (w232:T19)
                n131 = call <vilib>:"Add State(s) to Queue__jki_lib_state_machine.vi"("State(s) in Front (\"\")"="Data: Process Sweep" ("State(s) in Front (\"\")"), "State(s) in (\"\")"=w234) -> ("States Out"=w233:string)  [unwired: 13 in]
              }
              event User Event {
                n132 = event-data() -> ("measureOffset"=w236:T41)  [unwired: 1 in]
                n133 = local write "Method"("measureOffset" ("String")) -> ()
                n134 = Bundle By Name(cluster=w238, "Measure Offset"=w236) -> (w237:T19)
                n135 = local write "Measure Offset"(w236) -> ()
                n136 = call <vilib>:"Add State(s) to Queue__jki_lib_state_machine.vi"("State(s) in Front (\"\")"="DSP: Zero DAQ Offset\nData: Zero Amplitude\nDSP: Measure DAQ Offset\nData: Restore Amplitude" ("State(s) in Front (\"\")"), "State(s) in (\"\")"=w242) -> ("States Out"=w241:string)  [unwired: 13 in]
              }
              event User Event {
                n137 = event-data() -> ("Reset Phase"=w244:T42)  [unwired: 1 in]
                n138 = local write "Method"("zeroPhase" ("String")) -> ()
                n139 = Bundle By Name(cluster=w246, "Measure Offset"=w244) -> (w245:T19)
                n140 = local write "Reset Phase"(w244) -> ()
                n141 = call <vilib>:"Add State(s) to Queue__jki_lib_state_machine.vi"("State(s) in (\"\")"=w249) -> ("States Out"=w248:string)  [unwired: 14 in]
              }
              event User Event {
                w251 = "DAQ: AUTO" ("State(s) in Front (\"\")")
                n142 = event-data() -> ()  [unwired: 1 in, 5 out]
                n143 = local write "Method"("autoConfigureDAQ" ("String")) -> ()
                n144 = local write "Payload"(w251) -> ()
                n145 = call <vilib>:"Add State(s) to Queue__jki_lib_state_machine.vi"("State(s) in Front (\"\")"=w251, "State(s) in (\"\")"=w255) -> ("States Out"=w254:string)  [unwired: 13 in]
              }
              event User Event {
                # "#todo\n????"
                n146 = event-data() -> ("PreFilter"=w257:T43)  [unwired: 1 in, 4 out]
                n147 = local write "Payload"(w257) -> ()
                n148 = Unbundle By Name(w260) -> ("SMO"=w259:refnum<class "Instrument.DAQ.lvclass">)
                n149 = Bundle By Name(cluster=w259, "Prefilter"=w257) -> (w258:refnum<class "Instrument.DAQ.lvclass">)
                n150 = local write "Method"("setPreFilter" ("String")) -> ()
                n151 = Bundle By Name(cluster=w260, "SMO"=w258) -> (w261:T19)
                n152 = call <vilib>:"Add State(s) to Queue__jki_lib_state_machine.vi"("State(s) in Front (\"\")"="" ("State(s) in Front (\"\")"), "State(s) in (\"\")"=w265) -> ("States Out"=w264:string)  [unwired: 13 in]
              }
              event User Event {
                n153 = event-data() -> ("Amplitude Limit"=w267:T44)  [unwired: 1 in, 4 out]
                n154 = Unbundle By Name(w270) -> ("SMO"=w269:refnum<class "Instrument.DAQ.lvclass">)
                n155 = Bundle By Name(cluster=w269, "Amplitude Limit"=w267) -> (w268:refnum<class "Instrument.DAQ.lvclass">)
                n156 = local write "Method"("setAmplitudeLimit" ("String")) -> ()
                n157 = local write "Payload"(w267) -> ()
                n158 = Bundle By Name(cluster=w270, "SMO"=w268) -> (w271:T19)
                n159 = call <vilib>:"Add State(s) to Queue__jki_lib_state_machine.vi"("State(s) in Front (\"\")"="Data: Process AO Channels" ("State(s) in Front (\"\")"), "State(s) in (\"\")"=w275) -> ("States Out"=w274:string)  [unwired: 13 in]
              }
              event User Event {
                n160 = event-data() -> ("DC Limit"=w277:T45)  [unwired: 1 in, 4 out]
                n161 = Unbundle By Name(w280) -> ("SMO"=w279:refnum<class "Instrument.DAQ.lvclass">)
                n162 = Bundle By Name(cluster=w279, "DC Limit"=w277) -> (w278:refnum<class "Instrument.DAQ.lvclass">)
                n163 = local write "Method"("setDCLimit" ("String")) -> ()
                n164 = local write "Payload"(w277) -> ()
                n165 = Bundle By Name(cluster=w280, "SMO"=w278) -> (w281:T19)
                n166 = call <vilib>:"Add State(s) to Queue__jki_lib_state_machine.vi"("State(s) in Front (\"\")"="Data: Process AO Channels" ("State(s) in Front (\"\")"), "State(s) in (\"\")"=w285) -> ("States Out"=w284:string)  [unwired: 13 in]
              }
              event User Event {
                n167 = event-data() -> ("Duty Cycle"=w287:T46)  [unwired: 1 in, 4 out]
                n168 = Unbundle By Name(w290) -> ("SMO"=w289:refnum<class "Instrument.DAQ.lvclass">)
                n169 = Bundle By Name(cluster=w289, "Duty Cycle"=w287) -> (w288:refnum<class "Instrument.DAQ.lvclass">)
                n170 = local write "Method"("setDutyCycle" ("String")) -> ()
                n171 = local write "Payload"(w287) -> ()
                n172 = Bundle By Name(cluster=w290, "SMO"=w288) -> (w291:T19)
                n173 = call <vilib>:"Add State(s) to Queue__jki_lib_state_machine.vi"("State(s) in Front (\"\")"="Data: Process AO Channels" ("State(s) in Front (\"\")"), "State(s) in (\"\")"=w295) -> ("States Out"=w294:string)  [unwired: 13 in]
              }
              event User Event {
                n174 = event-data() -> ("Link Frequencies"=w297:T47)  [unwired: 1 in, 4 out]
                n175 = Unbundle By Name(w300) -> ("SMO"=w299:refnum<class "Instrument.DAQ.lvclass">)
                n176 = Bundle By Name(cluster=w299, "Link Frequencies"=w297) -> (w298:refnum<class "Instrument.DAQ.lvclass">)
                n177 = local write "Method"("setLinkFrequencies" ("String")) -> ()
                n178 = local write "Payload"(w297) -> ()
                n179 = Bundle By Name(cluster=w300, "SMO"=w298) -> (w301:T19)
                n180 = call <vilib>:"Add State(s) to Queue__jki_lib_state_machine.vi"("State(s) in Front (\"\")"="Data: Process AO Channels\nData: Process REF Channels" ("State(s) in Front (\"\")"), "State(s) in (\"\")"=w305) -> ("States Out"=w304:string)  [unwired: 13 in]
              }
              event User Event {
                n181 = event-data() -> ()  [unwired: 1 in, 5 out]
                n182 = local write "Method"("zeroOffset" ("String")) -> ()
                n183 = local write "Zero Offset"(TRUE ("zero offset")) -> ()
                n184 = call <vilib>:"Add State(s) to Queue__jki_lib_state_machine.vi"("State(s) in Front (\"\")"="DSP: Zero DAQ Offset" ("State(s) in Front (\"\")"), "State(s) in (\"\")"=w312) -> ("States Out"=w311:string)  [unwired: 13 in]
              }
              event User Event {
                # "start: Start acquisition (Macro: Acquire)\nstop: Stop acquisition (Macro: Stop)\nreset: Stop and Start acquisition (Macro: Stop, Macro: Start)\n\nif already running:\n- the private events setAOconfig, setAIconfig, setSampling\nwill be written to data cluster, but otherwise will be ignored until\nacquisition is reset\n- setAO and setREF will be implemented on next Acquisition iteration"
                n185 = event-data() -> ("setState"=w315:T48)  [unwired: 1 in]
                n186 = Unbundle By Name(w314) -> ("DAQ Status"=w316:T1)
                n187 = local write "Payload"(w315) -> ()
                n188 = local write "Method"("setState" ("String")) -> ()
                n189 = case shown="\"stop sweep\"" w315 {
                  tunnel: w316 -> [w322 _ w331 _ _]
                  tunnel: [w321 "Generator: Stop\nMacro: Stop DAQmx" ("State(s) in Front (\"\")") w327 w332 "Generator: Stop Sweep" ("format string")] -> w313
                  frame "start", Default {
                    n190 = case shown="Default" w322 {
                      tunnel: ["" ("State(s) in Front (\"\")") "Generator: Start\nMacro: Start DAQmx" ("State(s) in Front (\"\")")] -> w321
                      frame "created", "started" {
                      }
                      frame Default {
                      }
                    }
                  }
                  frame "stop" {
                  }
                  frame "reset" {
                    n191 = Equal?(x=Status--enum."idle" ("state"), y=w331) -> (x = y?=w330:bool)
                    n192 = Select(t="Data: Clear Sweep Data", s=w330, f="Macro: Stop DAQmx\nGenerator: Stop\nGenerator: Start\nMacro: Start DAQmx" ("State(s) in Front (\"\")")) -> (s? t:f=w327:string)
                    "reset" <- w327
                  }
                  frame "start sweep" {
                    w332 = "Sweep: Initialize\nData: Clear Sweep Data\nGenerator: Start Sweep" ("format string")
                    "start sweep" <- w332
                  }
                  frame "stop sweep" {
                  }
                }
                n193 = call <vilib>:"Add State(s) to Queue__jki_lib_state_machine.vi"("State(s) in (\"\")"=w320, "State(s) at Back (\"\")"=w313) -> ("States Out"=w319:string)  [unwired: 13 in]
              }
              event User Event {
                n194 = event-data() -> ("setCalibration"=w334:T14)  [unwired: 1 in, 4 out]
                n195 = local write "Method"("setCalibration" ("String")) -> ()
                n196 = local write "Payload"(w334) -> ()
                n197 = Format Into String(w334) -> (resulting string=w335:string)  [unwired: 3 in, 1 out]
                n198 = call <vilib>:"Build State String with Arguments__JKI_lib_State_Machine.vi"("Arguments (\"\")"=w335, "State"="DAQ: CALIBRATE" ("State(s) in Front (\"\")")) -> ("State with Arguments"=w338:string)  [unwired: 4 in]
                n199 = call <vilib>:"Add State(s) to Queue__jki_lib_state_machine.vi"("State(s) in (\"\")"=w342, "State(s) at Back (\"\")"=w338) -> ("States Out"=w341:string)  [unwired: 13 in]
              }
              event User Event {
                n200 = event-data() -> ("showDAQUI"=w347:T49)  [unwired: 1 in, 4 out]
                n201 = local write "Method"("showUI" ("String")) -> ()
                n202 = Select(t="Open", s=w347, f="Close") -> (s? t:f=w344:string)
                n203 = local write "Payload"(w344) -> ()
                n204 = call <vilib>:"Build State String with Arguments__JKI_lib_State_Machine.vi"("Arguments (\"\")"=w344, "State"="UI: Front Panel State" ("State(s) in Front (\"\")")) -> ("State with Arguments"=w343:string)  [unwired: 4 in]
                n205 = call <vilib>:"Add State(s) to Queue__jki_lib_state_machine.vi"("State(s) in Front (\"\")"=w343, "State(s) in (\"\")"=w353) -> ("States Out"=w352:string)  [unwired: 13 in]
              }
              event User Event {
                n206 = event-data() -> ("Status"=w354:T2)  [unwired: 1 in, 4 out]
                "DAQmx Status" <- w354
                n207 = local write "Method"("DAQmx.Status" ("String")) -> ()
                n208 = Bundle By Name(cluster=w358, "DAQmx Status"=w354) -> (w356:T19)
                n209 = call <vilib>:"Add State(s) to Queue__jki_lib_state_machine.vi"("State(s) in Front (\"\")"="Data: Process State >> -DAQmx" ("State(s) in Front (\"\")"), "State(s) in (\"\")"=w360) -> ("States Out"=w361:string)  [unwired: 13 in]
              }
              event User Event {
                n210 = event-data() -> ("Devices"=w362:T50[])  [unwired: 1 in, 4 out]
                n211 = local write "Payload"(w362) -> ()
                n212 = local write "Method"("DAQmx.Devices" ("String")) -> ()
                n213 = Unbundle By Name(w366) -> ("SMO"=w368:refnum<class "Instrument.DAQ.lvclass">)
                n214 = Bundle By Name(cluster=w368, "Devices"=w362) -> (w364:refnum<class "Instrument.DAQ.lvclass">)
                n215 = Bundle By Name(cluster=w366, "SMO"=w364) -> (w367:T19)
                n216 = call <vilib>:"Add State(s) to Queue__jki_lib_state_machine.vi"("State(s) in Front (\"\")"="Data: Process Devices >> -DAQmx" ("State(s) in Front (\"\")"), "State(s) in (\"\")"=w370) -> ("States Out"=w371:string)  [unwired: 13 in]
              }
              event User Event {
                n217 = event-data() -> ("Calibration out"=w372:T51)  [unwired: 1 in, 4 out]
                n218 = call "Convert DAQmx to DAQ cal.vi"("Calibration in"=w372) -> ("Array"=w373:T52[])  [unwired: 10 in]
                n219 = local write "Payload"(w372) -> ()
                n220 = local write "Method"("DAQmx.Calibration" ("String")) -> ()
                n221 = Unbundle By Name(w377) -> ("SMO"=w379:refnum<class "Instrument.DAQ.lvclass">)
                n222 = Bundle By Name(cluster=w379, "Calibration"=w373) -> (w374:refnum<class "Instrument.DAQ.lvclass">)
                n223 = Bundle By Name(cluster=w377, "SMO"=w374) -> (w378:T19)
                n224 = call <vilib>:"Add State(s) to Queue__jki_lib_state_machine.vi"("State(s) in Front (\"\")"="Data: Process Calibration >> -DAQmx" ("State(s) in Front (\"\")"), "State(s) in (\"\")"=w381) -> ("States Out"=w382:string)  [unwired: 13 in]
              }
              event User Event {
                n225 = event-data() -> ("Source"=w391:T53, "Sampling"=w383:T54, "sample mode"=w388:i32, "FsMode"=w384:T55, "Fs Multiplier"=w390:dbl, "Refresh Rate (Hz)"=w389:dbl, "Decimation.PreDSP"=w387:i32, "Fs.Output"=w386:dbl)  [unwired: 1 in, 4 out]
                n226 = local write "Method"("DAQmx.Timing" ("String")) -> ()
                n227 = Unbundle By Name(w393) -> ("SMO"=w395:refnum<class "Instrument.DAQ.lvclass">)
                n228 = Bundle By Name(cluster=w395, "Sampling"=w383, "sample mode"=w391, "Fs Mode"=w384, "Fs Multiplier"=w390, "Refresh Rate (Hz)"=w389, "Decimation.PreDSP"=w388, "Decimation.PostDSP"=w387, "Fs.Output"=w386) -> (w394:refnum<class "Instrument.DAQ.lvclass">)
                n229 = local write "Payload"(w383) -> ()
                n230 = Bundle By Name(cluster=w393, "SMO"=w394) -> (w392:T19)
                n231 = call <vilib>:"Add State(s) to Queue__jki_lib_state_machine.vi"("State(s) in Front (\"\")"="Data: Process Sampling >> -DAQmx" ("State(s) in Front (\"\")"), "State(s) in (\"\")"=w398) -> ("States Out"=w399:string)  [unwired: 13 in]
              }
              event User Event {
                n232 = event-data() -> ("AOconfig"=w400:T56)  [unwired: 1 in, 4 out]
                n233 = Unbundle By Name(w401) -> ("SMO"=w404:refnum<class "Instrument.DAQ.lvclass">)
                n234 = Bundle By Name(cluster=w404, "AO"=w400) -> (w403:refnum<class "Instrument.DAQ.lvclass">)
                n235 = local write "Method"("DAQmx.AOconfig" ("String")) -> ()
                n236 = local write "Payload"(w400) -> ()
                n237 = Bundle By Name(cluster=w401, "SMO"=w403) -> (w402:T19)
                n238 = call <vilib>:"Add State(s) to Queue__jki_lib_state_machine.vi"("State(s) in Front (\"\")"="Data: Process DAQ >> -DAQmx\nData: Process AO Channels >> -DAQmx" ("State(s) in Front (\"\")"), "State(s) in (\"\")"=w408) -> ("States Out"=w409:string)  [unwired: 13 in]
              }
              event User Event {
                n239 = event-data() -> ("AIconfig"=w410:T60)  [unwired: 1 in, 4 out]
                n240 = local write "Payload"(w410) -> ()
                n241 = Unbundle By Name(w412) -> ("SMO"=w415:refnum<class "Instrument.DAQ.lvclass">)
                n242 = Bundle By Name(cluster=w415, "AI"=w410) -> (w414:refnum<class "Instrument.DAQ.lvclass">)
                n243 = local write "Method"("DAQmx.AIconfig" ("String")) -> ()
                n244 = Bundle By Name(cluster=w412, "SMO"=w414) -> (w413:T19)
                n245 = call <vilib>:"Add State(s) to Queue__jki_lib_state_machine.vi"("State(s) in Front (\"\")"="Data: Process DAQ >> -DAQmx\nData: Process AI Channels >> -DAQmx" ("State(s) in Front (\"\")"), "State(s) in (\"\")"=w418) -> ("States Out"=w419:string)  [unwired: 13 in]
              }
              event User Event {
                n246 = event-data() -> ("AO"=w423:waveform(dbl)[], "AI"=w420:waveform(dbl)[], "REF_X"=w422:waveform(dbl)[], "REF_Y"=w421:waveform(dbl)[])  [unwired: 1 in, 4 out]
                n247 = Unbundle By Name(w432) -> ("SMO"=w429:refnum<class "Instrument.DAQ.lvclass">)
                n248 = local write "Method"("DAQmx.Waveforms" ("String")) -> ()
                n249 = call "Multiply Waveform by Output Gain.vi"("WFM in"=w423, "Instrument.DAQ"=w429) -> ("error out"=w425:errorcluster, "WFM out"=w430:waveform(dbl)[])  [unwired: 7 in, 1 out]
                n250 = call "Divide Waveform by Input Gain.vi"("WFM in"=w420, "Instrument.DAQ"=w429) -> ("error out"=w426:errorcluster, "WFM out"=w424:waveform(dbl)[])  [unwired: 7 in, 1 out]
                n251 = Bundle By Name(cluster=w429, "AO"=w430, "AI"=w424, "REF_X"=w422, "REF_Y"=w421) -> (w434:refnum<class "Instrument.DAQ.lvclass">)
                n252 = Merge Errors(w427, w426, w425) -> (w428:errorcluster)
                n253 = Bundle By Name(cluster=w432, "SMO"=w434) -> (w433:T19)
                n254 = call <vilib>:"Add State(s) to Queue__jki_lib_state_machine.vi"("State(s) in Front (\"\")"="Macro: DSP" ("State(s) in Front (\"\")"), "State(s) in (\"\")"=w436) -> ("States Out"=w437:string)  [unwired: 13 in]
              }
              event User Event {
                # "report sweeping when a sweep starts."
                n255 = event-data() -> ("sweep status"=w447:T13)  [unwired: 1 in]
                n256 = Format Into String(w447) -> (resulting string=→"sweep status":string)  [unwired: 3 in, 1 out]
                n257 = case shown="\"sweeping\"" w447 {
                  tunnel: [Status--enum."started" ("status") Status--enum."sweeping" ("status")] -> w441
                  frame Default {
                  }
                  frame "sweeping" {
                  }
                }
                n258 = local write "Method"("Generator.SweepState" ("String")) -> ()
                n259 = Unbundle By Name(w446) -> ("SMO"=w448:refnum<class "Instrument.DAQ.lvclass">)
                n260 = call "Is Value Changed.vim"("value"=w441) -> ("changed or first call?"=w439:bool)
                n261 = Equal?(x=w441, y=Status--enum."sweeping" ("status")) -> (x = y?=w440:bool)
                n262 = And(x=w439, y=w440) -> (x .and. y?=w438:bool)
                n263 = case shown="True" w438 {
                  tunnel: w448 -> [_ w457]
                  tunnel: w441 -> [_ w456]
                  tunnel: [w453 w455] -> w445
                  tunnel: w444 -> [w453 w454]
                  frame False {
                  }
                  frame True {
                    n264 = call "DAQ.getDAQState.vi"("error in (no error)"=w454, "status"=w456, "Instrument.DAQ"=w457) -> ("error out"=w455:errorcluster)  [unwired: 7 in, 1 out]
                  }
                }
                n265 = call <userlib>:"MGI Milliseconds Since Last Call.vi"() -> ("ms"=→"Generate (ms)" →"Generator Chart":u32)  [unwired: 6 in, 1 out]
                n266 = call <vilib>:"Add State(s) to Queue__jki_lib_state_machine.vi"("State(s) in (\"\")"=w451) -> ("States Out"=w450:string)  [unwired: 14 in]
              }
              event User Event {
                n267 = event-data() -> ("AO Channels"=w471:T64)  [unwired: 1 in, 4 out]
                n268 = Unbundle By Name(w468) -> ("SMO"=w470:refnum<class "Instrument.DAQ.lvclass">)
                n269 = local write "Method"("Generator.AOchannels" ("String")) -> ()
                n270 = call "Merge AO Settings from Generator.vi"("error in (no error)"=w467, "configuration.AO Channels"=w471, "Instrument.DAQ in"=w470) -> ("error out"=w461:errorcluster, "Instrument.DAQ out"=w463:refnum<class "Instrument.DAQ.lvclass">)  [unwired: 7 in]
                n271 = call "Multiply Amplitude and Offset by Output Gain.vi"("error in (no error)"=w461, "Instrument.DAQ"=w463) -> ("error out"=w460:errorcluster, "Instrument.DAQ out"=w462:refnum<class "Instrument.DAQ.lvclass">)  [unwired: 8 in]
                n272 = Bundle By Name(cluster=w468, "SMO"=w462) -> (w469:T19)
                n273 = call <vilib>:"Add State(s) to Queue__jki_lib_state_machine.vi"("State(s) in Front (\"\")"="Data: Update AO Channels" ("States Out"), "State(s) in (\"\")"=w465) -> ("States Out"=w466:string)  [unwired: 13 in]
              }
            }
          }
          frame "---------- Core ----------" {
            # "Do not put any code in this frame.\n(it is a separator no-op)"
            n274 = call <vilib>:"Add State(s) to Queue__jki_lib_state_machine.vi"("State(s) in (\"\")"=w477) -> ("States Out"=w476:string)  [unwired: 14 in]
          }
          frame Default {
            w488 = 42 items=["No error", "Argument error", "Memory is full", "Out of zone", "End of file", "File already open", "Generic file I/O error", "File not found", "File permission error", "Disk is full", "Duplicate path", "Too many files open", "System feature not enabled", "Resource file not found", "Cannot add resource", "Resource not found", "Image not found", "Image memory error", "Pen does not exist", "Config type invalid", "Config token not found", "Config parse error", "Config memory error", "Bad external code format", "Bad external code offset", "External code not present", "Null window", "Destroy window error", "Null menu", "Print aborted", "Bad print record", "Print driver error", "Windows error during printing", "Memory error during printing", "Print dialog error", "Generic print error", "Invalid device refnum", "Device not found", "Device parameter error", "Device unit error", "Cannot open device", "Device call aborted", "Generic error", "Cancelled by user", "Object ID too low", "Object ID too high", "Object not in heap", "Unknown heap", "Unknown object (invalid DefProc)", "Unknown object (DefProc not in table)", "Message out of range", "Invalid (null) method", "Unknown message", "Manager call not supported", "Bad address", "Network operation in progress", "Network operation timed out", "Connection is busy", "Network attribute not supported", "Network error", "Address in use", "System out of memory", "Connection aborted", "Connection refused", "Not connected", "Already connected", "Connection closed", "Initialization error (interapplication manager)", "Bad occurrence", "Wait on unbound occurrence handler", "Occurrence queue overflow", "Datalog type conflict", "Unused", "Unrecognized type (interapplication manager)", "Memory corrupt", "Failed to make temporary DLL", "Old CIN version", "Drag socket not found", "Failed to load drop-object", "Failed to register OLE object", "Failed to release OLE object", "Format specifier type mismatch", "Unknown format specifier", "Too few format specifiers", "Too many format specifiers", "Scan failed", "Newer CIN version", "Error converting to variant", "Runtime menu error", "Password tampered", "Variant attribute not found", "Incompatible variant data type", "Event data is not available", "Event Store is not present", "Occurrence is not found", "Event Queue is not created", "Event info is not available", "Refnum passed is NULL", "Error retrieving Class GUID", "Error retrieving CoClass GUID", "Error retrieving TypeLib GUID.", "Bad built application magic bytes.", "Specific driver is different from the specific driver associated with the Logical Name.", "There is no session opened to the class driver.", "Max Error", "MAX - Error with config objects", "MAX - Error loading configuration", "MAX - Group not supported"]
            # "Current State"
            # "Do not delete, rename, or modify this frame.\n(this is used to capture unhandled states and typos)"
            # "Handle mistyped state name (developer tool)"
            n275 = Format Into String(format string="Software Exception: Unhandled State \"%s\"." ("message"), error in=w484, w479) -> (resulting string=w487:string, error out=w486:errorcluster)  [unwired: 1 in]
            n276 = call <vilib>:"Error Cluster From Error Code.vi"("show call chain? (False)"=TRUE, "error in (no error)"=w486, "error message (\"\")"=w487, "error code (0)"=w488) -> ("error out"=w485:errorcluster)  [unwired: 5 in]
            n277 = call <vilib>:"Add State(s) to Queue__jki_lib_state_machine.vi"("State(s) in (\"\")"=w483) -> ("States Out"=w482:string)  [unwired: 14 in]
          }
          frame "Initialize Core Data" {
            # "Do not delete, rename, or modify this frame.\n(this is used to determine panel behavior on exit)"
            # "originally closed?"
            # "exe?"
            # "If panel starts closed or is an EXE, then close it when we exit"
            n278 = property class="VI"() -> ("Front Panel.Open"=w498:bool)  [unwired: 2 in, 2 out]
            n279 = property class="App"() -> ("App.Kind"=w497:T10)  [unwired: 2 in, 2 out]
            n280 = control-ref of="Current VI Reference"() -> (w491:refnum<vi>)
            n281 = Not(x=w498) -> (.not. x?=w495:bool)
            n282 = Equal?(x=w497, y=T10."Run Time System" ("Application:Kind")) -> (x = y?=w494:bool)
            n283 = Or(x=w495, y=w494) -> (x .or. y?=w492:bool)
            n284 = Bundle By Name(cluster=w493, "Core.Current VI Reference"=w491, "Core.Close Panel on Exit?"=w492) -> (w500:T19)
            n285 = call <vilib>:"Add State(s) to Queue__jki_lib_state_machine.vi"("State(s) in (\"\")"=w502) -> ("States Out"=w501:string)  [unwired: 14 in]
          }
          frame "Error Handler" {
            w509 = FALSE  # Stop on Unhandled Error (T)
            # "Clear error"
            # "There was an error while handling the error.\nStop the process. This error can only occur if public events references are invalid or if the state machine object is destroyed."
            n286 = Unbundle By Name(w513) -> ("SMO"=w506:refnum<class "Instrument.DAQ.lvclass">)
            n287 = call-dynamic "Handle Error.vi"("Stop on Unhandled Error (T)"=w509, "error in"=w505, "SMO"=w506) -> ("handling error"=w510:errorcluster, "Unhandled error"=w507:errorcluster)  [unwired: 6 in, 1 out]
            n288 = Bundle By Name(cluster=w513, "Core.Last Error.remaining states"=w504, "Core.Last Error.error"=w507) -> (w512:T19)
            n289 = Select(t="Exit", s=w510, f="Macro: Post Error Handling") -> (s? t:f=w508:string)
          }
          frame "Exit" {
            # "Do not put any code in this frame.\n(No errors that occur here will be handled.)"
            n290 = Unbundle By Name(w517) -> ("Core.Last Error.error"=w516:errorcluster)
            n291 = call <vilib>:"Add State(s) to Queue__jki_lib_state_machine.vi"("State(s) in (\"\")"=w521) -> ("States Out"=w520:string)  [unwired: 14 in]
          }
          frame "---------- Data ----------" {
            # "Do not put any code in this frame.\n(It is a separator no-op. You can make a copy of this frame to create a new Data frame)"
            n292 = call <vilib>:"Add State(s) to Queue__jki_lib_state_machine.vi"("State(s) in (\"\")"=w526) -> ("States Out"=w525:string)  [unwired: 14 in]
          }
          frame "Data: Initialize" {
            w527 = Generator.Sweep_Status--enum."stopping"  # Sweep Status
            w528 = dbl[] []  # Saved Amplitudes
            w529 = DAQmx.Status--enum."idle"  # DAQmx Status
            w532 = T67 {"Current VI Reference"=refnum, "Close Panel on Exit?"=FALSE, "Last Error"={"error"={"status"=FALSE, "code"=0, "source"=""}, "previous state"="", "remaining states"=""}, "Shutdown?"=FALSE}  # Core
            w531 = T11 {"AO"=[], "AI"=[], "X"=[], "Y"=[]}  # SweepWaveforms
            w535 = FALSE  # Measure Offset
            w530 = T18 {"Time Stamp"=timestamp(0 s since 1904-01-01), "Results (Dictionary)"=[]}  # Results
            w537 = Status--enum."idle"  # DAQ Status
            # "starts in idle mode"
            # "Initialize the shift-register data, here.\n(data names are defined by what you wire into the bundle function)"
            n293 = local write "Status"(w537) -> ()
            n294 = call "DAQ.getDAQState.vi"("error in (no error)"=w534, "status"=w537, "Instrument.DAQ"=w533) -> ("error out"=w536:errorcluster)  [unwired: 7 in, 1 out]
            n295 = call <vilib>:"Add State(s) to Queue__jki_lib_state_machine.vi"("State(s) in (\"\")"=w541) -> ("States Out"=w540:string)  [unwired: 14 in]
            n296 = Bundle("Core"=w532, "SMO"=w533, "DAQ Status"=w537, "DAQmx Status"=w529, "Sweep Status"=w527, "Results"=w530, "SweepWaveforms"=w531, "Measure Offset"=w535, "Saved Amplitudes"=w528) -> (w538:T19)  [unwired: 1 in]
          }
          frame "Data: Process State" {
            # "Data: Process State.\n()"
            n297 = Unbundle By Name(w546) -> ("DAQmx Status"=w544:T2)
            n298 = case shown="\"clearing\"" w544 {
              tunnel: [Status--enum."idle" ("state") Status--enum."idle" ("state") Status--enum."idle" ("state") Status--enum."idle" ("state") Status--enum."created" ("state") Status--enum."created" ("state") Status--enum."started" ("state") Status--enum."started" ("state") Status--enum."stopped" ("state") Status--enum."idle" ("state") Status--enum."idle" ("state")] -> w542
              frame "idle", Default {
              }
              frame "calibrating" {
              }
              frame "configuring" {
              }
              frame "creating" {
              }
              frame "created" {
              }
              frame "starting" {
              }
              frame "started" {
              }
              frame "stopping" {
              }
              frame "stopped" {
              }
              frame "clearing" {
              }
              frame "error" {
              }
            }
            "Status" <- w542
            n299 = Unbundle By Name(w546) -> ("SMO"=w549:refnum<class "Instrument.DAQ.lvclass">)
            n300 = call "DAQ.getDAQState.vi"("error in (no error)"=w547, "status"=w542, "Instrument.DAQ"=w549) -> ("error out"=w543:errorcluster, "Instrument.DAQ out"=w545:refnum<class "Instrument.DAQ.lvclass">)  [unwired: 7 in]
            n301 = Bundle By Name(cluster=w546, "SMO"=w545, "DAQ Status"=w542) -> (w548:T19)
            n302 = call <vilib>:"Add State(s) to Queue__jki_lib_state_machine.vi"("State(s) in (\"\")"=w552) -> ("States Out"=w551:string)  [unwired: 14 in]
          }
          frame "Data: Process Devices" {
            # "Data: Process Devices.\n()"
            n303 = Unbundle By Name(w568) -> ("SMO"=w567:refnum<class "Instrument.DAQ.lvclass">)
            n304 = Unbundle By Name(w567) -> ("Devices"=w564:T68[])
            n305 = call "DAQ.getDeviceIDN.vi"("error in (no error)"=w565, "Devices"=w564, "Instrument.DAQ"=w567) -> ("error out"=w566:errorcluster, "Instrument.DAQ out"=w570:refnum<class "Instrument.DAQ.lvclass">)  [unwired: 7 in]
            n306 = Bundle By Name(cluster=w568, "SMO"=w570) -> (w569:T19)
            n307 = call <vilib>:"Add State(s) to Queue__jki_lib_state_machine.vi"("State(s) in (\"\")"=w573) -> ("States Out"=w572:string)  [unwired: 14 in]
          }
          frame "Data: Process Calibration" {
            # "Data: Process Calibration.\n()"
            n308 = Unbundle By Name(w574) -> ("SMO"=w578:refnum<class "Instrument.DAQ.lvclass">)
            n309 = Unbundle By Name(w578) -> ("Calibration"=w579:T69)
            n310 = call "DAQ.getCalibration.vi"("error in (no error)"=w576, "Calibration"=w579, "Instrument.DAQ"=w578) -> ("error out"=w577:errorcluster, "Instrument.DAQ"=w580:refnum<class "Instrument.DAQ.lvclass">)  [unwired: 7 in]
            n311 = Bundle By Name(cluster=w574, "SMO"=w580) -> (w575:T19)
            n312 = call <vilib>:"Add State(s) to Queue__jki_lib_state_machine.vi"("State(s) in (\"\")"=w583) -> ("States Out"=w582:string)  [unwired: 14 in]
          }
          frame "Data: Process DAQ" {
            # "Data: Process DAQ.\n()"
            n313 = Unbundle By Name(w595) -> ("SMO"=w593:refnum<class "Instrument.DAQ.lvclass">)
            n314 = Unbundle By Name(w593) -> ("DAQmx"=w591:refnum<class "DAQmx.lvclass">, "AI"=w589:T23, "AO"=w590:T20)
            n315 = call "config not UI to UI (AO and AI).vi"("error in (no error)"=w588, "AO Config"=w590, "AI Config"=w589) -> ("error out"=w587:errorcluster, "New Ch []"=w594:T70)  [unwired: 7 in]
            n316 = call "DAQ.getDAQconfig.vi"("error in (no error)"=w587, "New Ch []"=w594, "Instrument.DAQ"=w593) -> ("error out"=w586:errorcluster, "Instrument.DAQ out"=w592:refnum<class "Instrument.DAQ.lvclass">)  [unwired: 7 in]
            n317 = case shown="Default" w584 {
              tunnel: w591 -> [_ w607]
              tunnel: w590 -> [_ w605]
              tunnel: w589 -> [_ w604]
              tunnel: w586 -> [w600 w603]
              tunnel: [w600 w601] -> w585
              frame "-DAQmx" {
              }
              frame Default {
                n318 = call "setAIconfig.vi"("error in (no error)"=w603, "AIconfig"=w604, "DAQmx in"=w607) -> ("error out"=w602:errorcluster, "DAQmx out"=w606:refnum<class "DAQmx.lvclass">)  [unwired: 7 in]
                n319 = call "setAOconfig.vi"("error in (no error)"=w602, "AOconfig"=w605, "DAQmx in"=w606) -> ("error out"=w601:errorcluster)  [unwired: 7 in, 1 out]
              }
            }
            n320 = Bundle By Name(cluster=w595, "SMO"=w592) -> (w596:T19)
            n321 = call <vilib>:"Add State(s) to Queue__jki_lib_state_machine.vi"("State(s) in (\"\")"=w599) -> ("States Out"=w598:string)  [unwired: 14 in]
          }
          frame "Data: Process Sampling" {
            # "Data: Process Sampling.\n(Preprocess Sampling)"
            n322 = Unbundle By Name(w624) -> ("SMO"=w623:refnum<class "Instrument.DAQ.lvclass">)
            n323 = Unbundle By Name(w623) -> ("DSP"=w617:refnum<class "DSP.lvclass">, "Generator"=w612:refnum<class "Generator.lvclass">)
            n324 = Unbundle By Name(w623) -> ("DAQmx"=w622:refnum<class "DAQmx.lvclass">, "Sampling"=w608:T34)
            n325 = call "DAQ.getSampling.vi"("error in (no error)"=w614, "Sampling"=w608, "Instrument.DAQ"=w623) -> ("error out"=w616:errorcluster, "Instrument.DAQ out"=w619:refnum<class "Instrument.DAQ.lvclass">)  [unwired: 7 in]
            n326 = call "Write Timing.vi"("error in (no error)"=w616, "Timing"=w608, "DSP in"=w617) -> ("error out"=w615:errorcluster, "DSP out"=w620:refnum<class "DSP.lvclass">)  [unwired: 7 in]
            n327 = Bundle By Name(cluster=w619, "DSP"=w620) -> (w618:refnum<class "Instrument.DAQ.lvclass">)
            n328 = case shown="Default" w621 {
              tunnel: w622 -> [_ w633]
              tunnel: w608 -> [_ w632]
              tunnel: w615 -> [w629 w631]
              tunnel: [w629 w630] -> w611
              frame "-DAQmx" {
              }
              frame Default {
                n329 = call "setTiming.vi"("error in (no error)"=w631, "Timing"=w632, "DAQmx in"=w633) -> ("error out"=w630:errorcluster)  [unwired: 7 in, 1 out]
              }
            }
            n330 = Unbundle By Name(w608) -> ("Sampling"=w609:T35)
            n331 = call "setSampling.vi"("error in (no error)"=w611, "Sampling"=w609, "Generator in"=w612) -> ("error out"=w610:errorcluster)  [unwired: 7 in, 1 out]
            n332 = Bundle By Name(cluster=w624, "SMO"=w618) -> (w625:T19)
            n333 = call <vilib>:"Add State(s) to Queue__jki_lib_state_machine.vi"("State(s) in Front (\"\")"="" ("f"), "State(s) in (\"\")"=w628) -> ("States Out"=w627:string)  [unwired: 13 in]
          }
          frame "Data: Process AI Channels" {
            # "Data: Process AI Channels.\n()"
            n334 = Unbundle By Name(w645) -> ("SMO"=w644:refnum<class "Instrument.DAQ.lvclass">)
            n335 = call "Initialize AI Channels.vi"("error in (no error)"=w642, "Instrument.DAQ"=w644) -> ("error out"=w643:errorcluster, "Instrument.DAQ out"=w641:refnum<class "Instrument.DAQ.lvclass">)  [unwired: 8 in]
            n336 = Unbundle By Name(w641) -> ("Cfg_AI"=w634:T30)
            n337 = Unbundle By Name(w641) -> ("DSP"=w640:refnum<class "DSP.lvclass">)
            n338 = call "DAQ.getAIChannels.vi"("error in (no error)"=w643, "Channels.AI"=w634, "Instrument.DAQ"=w641) -> ("error out"=w638:errorcluster, "Instrument.DAQ out"=w636:refnum<class "Instrument.DAQ.lvclass">)  [unwired: 7 in]
            n339 = call "Write AI Channels.vi"("error in (no error)"=w638, "AI Channels"=w634, "DSP in"=w640) -> ("error out"=w637:errorcluster, "DSP out"=w639:refnum<class "DSP.lvclass">)  [unwired: 7 in]
            n340 = Bundle By Name(cluster=w636, "DSP"=w639) -> (w635:refnum<class "Instrument.DAQ.lvclass">)
            n341 = Bundle By Name(cluster=w645, "SMO"=w635) -> (w646:T19)
            n342 = call <vilib>:"Add State(s) to Queue__jki_lib_state_machine.vi"("State(s) in (\"\")"=w649) -> ("States Out"=w648:string)  [unwired: 14 in]
          }
          frame "Data: Process AO Channels" {
            # "Data: Process AO Channels.\n()"
            n343 = Unbundle By Name(w670) -> ("SMO"=w669:refnum<class "Instrument.DAQ.lvclass">)
            n344 = call "Initialize AO Channels.vi"("error in (no error)"=w668, "Instrument.DAQ"=w669) -> ("error out"=w662:errorcluster, "Instrument.DAQ out"=w667:refnum<class "Instrument.DAQ.lvclass">)  [unwired: 8 in]
            n345 = call "Limit AO Amplitude.vi"("error in (no error)"=w662, "Instrument.DAQ"=w667) -> ("error out"=w660:errorcluster, "Instrument.DAQ out"=w665:refnum<class "Instrument.DAQ.lvclass">)  [unwired: 8 in]
            n346 = call "Limit AO DC.vi"("error in (no error)"=w660, "Instrument.DAQ"=w665) -> ("error out"=w659:errorcluster, "Instrument.DAQ out"=w664:refnum<class "Instrument.DAQ.lvclass">)  [unwired: 8 in]
            n347 = call "Set all f same.vi"("error in (no error)"=w659, "Instrument.DAQ"=w664) -> ("error out"=w651:errorcluster, "Instrument.DAQ out"=w653:refnum<class "Instrument.DAQ.lvclass">)  [unwired: 8 in]
            n348 = Unbundle By Name(w653) -> ("Cfg_AO"=w663:T27)
            n349 = call "Divide Amplitude and Offset by Output Gain.vi"("error in (no error)"=w651, "Instrument.DAQ"=w653) -> ("error out"=w650:errorcluster, "Instrument.DAQ out"=w652:refnum<class "Instrument.DAQ.lvclass">)  [unwired: 8 in]
            n350 = call "Merge AO Settings to Generator.vi"("error in (no error)"=w650, "Instrument.DAQ in"=w652) -> ("error out"=w658:errorcluster, "AO Channels"=w654:T64, "Instrument.DAQ out"=w655:refnum<class "Instrument.DAQ.lvclass">)  [unwired: 7 in]
            n351 = Unbundle By Name(w655) -> ("Generator"=w656:refnum<class "Generator.lvclass">)
            n352 = call "setAOChannels.vi"("error in (no error)"=w658, "AO Channels"=w654, "Generator in"=w656) -> ("error out"=w657:errorcluster)  [unwired: 7 in, 1 out]
            n353 = call "DAQ.getAOChannels.vi"("error in (no error)"=w657, "Channels: AO"=w663, "Instrument.DAQ"=w653) -> ("error out"=w661:errorcluster, "Instrument.DAQ out"=w666:refnum<class "Instrument.DAQ.lvclass">)  [unwired: 7 in]
            n354 = Bundle By Name(cluster=w670, "SMO"=w666) -> (w671:T19)
            n355 = call <vilib>:"Add State(s) to Queue__jki_lib_state_machine.vi"("State(s) in (\"\")"=w674) -> ("States Out"=w673:string)  [unwired: 14 in]
          }
          frame "Data: Process REF Channels" {
            # "Data: Process REF Channels.\n()"
            n356 = Unbundle By Name(w690) -> ("SMO"=w688:refnum<class "Instrument.DAQ.lvclass">)
            n357 = call "Initialize REF Channels.vi"("error in (no error)"=w689, "Instrument.DAQ"=w688) -> ("error out"=w687:errorcluster, "Instrument.DAQ out"=w685:refnum<class "Instrument.DAQ.lvclass">)  [unwired: 8 in]
            n358 = call "Set all f same.vi"("error in (no error)"=w687, "Instrument.DAQ"=w685) -> ("error out"=w686:errorcluster, "Instrument.DAQ out"=w684:refnum<class "Instrument.DAQ.lvclass">)  [unwired: 8 in]
            n359 = Unbundle By Name(w684) -> ("Cfg_REF"=w678:T32)
            n360 = Unbundle By Name(w684) -> ("DSP"=w683:refnum<class "DSP.lvclass">, "Generator"=w677:refnum<class "Generator.lvclass">)
            n361 = call "DAQ.getREFChannels.vi"("error in (no error)"=w686, "Channels.REF"=w678, "Instrument.DAQ"=w684) -> ("error out"=w679:errorcluster, "Instrument.DAQ out"=w682:refnum<class "Instrument.DAQ.lvclass">)  [unwired: 7 in]
            n362 = call "Write REF Channels.vi"("error in (no error)"=w679, "REF Channels"=w678, "DSP in"=w683) -> ("error out"=w676:errorcluster, "DSP out"=w680:refnum<class "DSP.lvclass">)  [unwired: 7 in]
            n363 = Bundle By Name(cluster=w682, "DSP"=w680) -> (w681:refnum<class "Instrument.DAQ.lvclass">)
            n364 = call "setREFChannels.vi"("error in (no error)"=w676, "REF Channels"=w678, "Generator in"=w677) -> ("error out"=w675:errorcluster)  [unwired: 7 in, 1 out]
            n365 = Bundle By Name(cluster=w690, "SMO"=w681) -> (w691:T19)
            n366 = call <vilib>:"Add State(s) to Queue__jki_lib_state_machine.vi"("State(s) in (\"\")"=w694) -> ("States Out"=w693:string)  [unwired: 14 in]
          }
          frame "Data: Process Input Gain" {
            # "Do not put any code in this frame.\n(It is a separator no-op. You can make a copy of this frame to create a new Data frame)"
            n367 = Unbundle By Name(w701) -> ("SMO"=w703:refnum<class "Instrument.DAQ.lvclass">)
            n368 = call "Initialize Input Gain.vi"("error in (no error)"=w697, "Instrument.DAQ"=w703) -> ("error out"=w699:errorcluster, "Input Gain"=w695:T72, "Instrument.DAQ out"=w700:refnum<class "Instrument.DAQ.lvclass">)  [unwired: 7 in]
            n369 = call "DAQ.getInputGain.vi"("error in (no error)"=w699, "Input Gain"=w695, "Instrument.DAQ"=w700) -> ("error out"=w696:errorcluster, "Instrument.DAQ out"=w698:refnum<class "Instrument.DAQ.lvclass">)  [unwired: 7 in]
            n370 = Bundle By Name(cluster=w701, "SMO"=w698) -> (w702:T19)
            n371 = call <vilib>:"Add State(s) to Queue__jki_lib_state_machine.vi"("State(s) in (\"\")"=w706) -> ("States Out"=w705:string)  [unwired: 14 in]
          }
          frame "Data: Process Input Offset" {
            # "Do not put any code in this frame.\n(It is a separator no-op. You can make a copy of this frame to create a new Data frame)"
            n372 = Unbundle By Name(w714) -> ("SMO"=w711:refnum<class "Instrument.DAQ.lvclass">)
            n373 = call "Initialize Input Offset.vi"("error in (no error)"=w708, "Instrument.DAQ"=w711) -> ("error out"=w707:errorcluster, "Offset out"=w710:T72, "Instrument.DAQ out"=w709:refnum<class "Instrument.DAQ.lvclass">)  [unwired: 7 in]
            n374 = call "DAQ.getInputOffset.vi"("error in (no error)"=w707, "Input Offset"=w710, "Instrument.DAQ"=w709) -> ("error out"=w712:errorcluster, "Instrument.DAQ out"=w713:refnum<class "Instrument.DAQ.lvclass">)  [unwired: 7 in]
            n375 = Bundle By Name(cluster=w714, "SMO"=w713) -> (w715:T19)
            n376 = call <vilib>:"Add State(s) to Queue__jki_lib_state_machine.vi"("State(s) in (\"\")"=w718) -> ("States Out"=w717:string)  [unwired: 14 in]
          }
          frame "Data: Process Output Gain" {
            # "Do not put any code in this frame.\n(It is a separator no-op. You can make a copy of this frame to create a new Data frame)"
            n377 = Unbundle By Name(w725) -> ("SMO"=w727:refnum<class "Instrument.DAQ.lvclass">)
            n378 = call "Initialize Ouput Gain.vi"("error in (no error)"=w720, "Instrument.DAQ"=w727) -> ("error out"=w722:errorcluster, "Output Gain"=w719:T72, "Instrument.DAQ out"=w724:refnum<class "Instrument.DAQ.lvclass">)  [unwired: 7 in]
            n379 = call "DAQ.getOutputGain.vi"("error in (no error)"=w722, "Output Gain"=w719, "Instrument.DAQ"=w724) -> ("error out"=w721:errorcluster, "Instrument.DAQ out"=w723:refnum<class "Instrument.DAQ.lvclass">)  [unwired: 7 in]
            n380 = Bundle By Name(cluster=w725, "SMO"=w723) -> (w726:T19)
            n381 = call <vilib>:"Add State(s) to Queue__jki_lib_state_machine.vi"("State(s) in (\"\")"=w730) -> ("States Out"=w729:string)  [unwired: 14 in]
          }
          frame "Data: Process Sweep" {
            # "Do any necessary pre-processing here"
            # "Do not put any code in this frame.\n(It is a separator no-op. You can make a copy of this frame to create a new Data frame)"
            n382 = Unbundle By Name(w743) -> ("SMO"=w742:refnum<class "Instrument.DAQ.lvclass">)
            n383 = call "Initialize Sweep Channels.vi"("error in (no error)"=w741, "Instrument.DAQ"=w742) -> ("error out"=w734:errorcluster, "Instrument.DAQ out"=w735:refnum<class "Instrument.DAQ.lvclass">)  [unwired: 8 in]
            n384 = Unbundle By Name(w735) -> ("Sweep"=w736:T37)
            n385 = call "DAQ.getSweepChannels.vi"("error in (no error)"=w734, "Channels.Sweep"=w736, "Instrument.DAQ"=w735) -> ("error out"=w731:errorcluster, "Instrument.DAQ out"=w733:refnum<class "Instrument.DAQ.lvclass">)  [unwired: 7 in]
            n386 = Unbundle By Name(w733) -> ("Generator"=w739:refnum<class "Generator.lvclass">)
            n387 = call "Divide Sweep Config by Output Gain.vi"("error in (no error)"=w731, "Instrument.DAQ"=w733) -> ("error out"=w732:errorcluster, "Instrument.DAQ out"=w738:refnum<class "Instrument.DAQ.lvclass">)  [unwired: 8 in]
            n388 = Unbundle By Name(w738) -> ("Sweep"=w737:T37)
            n389 = call "setSweepChannels.vi"("error in (no error)"=w732, "Sweep Channels"=w737, "Generator in"=w739) -> ("error out"=w740:errorcluster)  [unwired: 7 in, 1 out]
            n390 = Bundle By Name(cluster=w743, "SMO"=w733) -> (w744:T19)
            n391 = call <vilib>:"Add State(s) to Queue__jki_lib_state_machine.vi"("State(s) in (\"\")"=w747) -> ("States Out"=w746:string)  [unwired: 14 in]
          }
          frame "Data: Update AO Channels" {
            n392 = Unbundle By Name(w752) -> ("SMO"=w751:refnum<class "Instrument.DAQ.lvclass">)
            n393 = Unbundle By Name(w751) -> ("Cfg_AO"=w753:T27)
            n394 = call "Is Value Changed.vim"("value"=w753) -> ("changed or first call?"=w750:bool)
            n395 = case shown="True" w750 {
              tunnel: w753 -> [_ w761]
              tunnel: w751 -> [_ w760]
              tunnel: [w757 w758] -> w749
              tunnel: w748 -> [w757 w759]
              frame False {
              }
              frame True {
                n396 = call "DAQ.getAOChannels.vi"("error in (no error)"=w759, "Channels: AO"=w761, "Instrument.DAQ"=w760) -> ("error out"=w758:errorcluster)  [unwired: 7 in, 1 out]
              }
            }
            n397 = call <vilib>:"Add State(s) to Queue__jki_lib_state_machine.vi"("State(s) in (\"\")"=w756) -> ("States Out"=w755:string)  [unwired: 14 in]
          }
          frame "Data: Zero Amplitude" {
            n398 = Unbundle By Name(w765) -> ("SMO"=w768:refnum<class "Instrument.DAQ.lvclass">)
            n399 = call "Zero AO Amplitudes.vi"("error in (no error)"=w763, "Instrument.DAQ in"=w768) -> ("error out"=w764:errorcluster, "Saved Amplitudes"=w762:dbl[], "Instrument.DAQ out"=w767:refnum<class "Instrument.DAQ.lvclass">)  [unwired: 7 in]
            n400 = Bundle By Name(cluster=w765, "SMO"=w767, "Saved Amplitudes"=w762) -> (w766:T19)
            n401 = call <vilib>:"Add State(s) to Queue__jki_lib_state_machine.vi"("State(s) in (\"\")"=w771) -> ("States Out"=w770:string)  [unwired: 14 in]
          }
          frame "Data: Restore Amplitude" {
            n402 = Unbundle By Name(w777) -> ("SMO"=w773:refnum<class "Instrument.DAQ.lvclass">, "Saved Amplitudes"=w776:dbl[])
            n403 = call "Restore AO Amplitudes.vi"("error in (no error)"=w775, "Saved Amplitudes"=w776, "Instrument.DAQ in"=w773) -> ("error out"=w774:errorcluster, "Instrument.DAQ out"=w772:refnum<class "Instrument.DAQ.lvclass">)  [unwired: 7 in]
            n404 = Bundle By Name(cluster=w777, "SMO"=w772) -> (w778:T19)
            n405 = call <vilib>:"Add State(s) to Queue__jki_lib_state_machine.vi"("State(s) in (\"\")"=w781) -> ("States Out"=w780:string)  [unwired: 14 in]
          }
          frame "Data: Clear Sweep Data" {
            w784 = waveform(dbl)[] [] ("X")
            n406 = Unbundle By Name(w789) -> ("SMO"=w788:refnum<class "Instrument.DAQ.lvclass">)
            n407 = Bundle By Name(cluster=T11 {"AO"=[], "AI"=[], "X"=[], "Y"=[]} ("SweepWFMs"), "AO"=w784, "AI"=w784, "X"=w784, "Y"=w784) -> (w782:T11)
            n408 = call "DAQ.getSweepWaveforms.vi"("error in (no error)"=w787, "SweepWFMs"=w782, "Instrument.DAQ"=w788) -> ("error out"=w785:errorcluster, "Instrument.DAQ out"=w786:refnum<class "Instrument.DAQ.lvclass">)  [unwired: 7 in]
            n409 = Bundle By Name(cluster=w789, "SMO"=w786, "SweepWaveforms"=w782) -> (w790:T19)
            n410 = call <vilib>:"Add State(s) to Queue__jki_lib_state_machine.vi"("State(s) in (\"\")"=w793) -> ("States Out"=w792:string)  [unwired: 14 in]
          }
          frame "Data: Save Sweep Data" {
            # "publish intermediate waveform"
            n411 = Unbundle By Name(w813) -> ("SweepWaveforms"=w811:T11)
            n412 = Unbundle By Name(w813) -> ("SMO"=w806:refnum<class "Instrument.DAQ.lvclass">)
            n413 = Unbundle By Name(w806) -> ("AO"=w810:waveform(dbl)[], "AI"=w809:waveform(dbl)[], "X"=w808:waveform(dbl)[], "Y"=w807:waveform(dbl)[])
            n414 = flat-sequence {
              tunnel: [w829] -> w799
              tunnel: w804 -> [w828]
              tunnel: [w828] -> w800
              frame #0 {
                n415 = call <vilib>:"High Resolution Relative Seconds.vi"() -> ("relative seconds"=w829:dbl)
              }
            }
            n416 = Bundle By Name(cluster=T11 {"AO"=[], "AI"=[], "X"=[], "Y"=[]} ("SweepWFMs"), "AO"=w810, "AI"=w809, "X"=w808, "Y"=w807) -> (w805:T11)
            n417 = call "DAQ.getSweepWaveforms.vi"("error in (no error)"=w800, "SweepWFMs"=w805, "Instrument.DAQ"=w806) -> ("Instrument.DAQ out"=w798:refnum<class "Instrument.DAQ.lvclass">)  [unwired: 7 in, 1 out]
            n418 = call "Append Sweep Waveforms.vi"("error in (no error)"=w800, "New SweepWaveforms"=w805, "SweepWaveforms in"=w811) -> ("error out"=w796:errorcluster, "SweepWaveforms out"=w794:T11)  [unwired: 7 in]
            n419 = case shown="\"final\"" w795 {
              tunnel: w798 -> [_ w823]
              tunnel: w794 -> [_ w822]
              tunnel: [w818 w825] -> w797
              tunnel: w796 -> [w818 w820]
              frame Default {
              }
              frame "final" {
                n420 = call "DAQ.getDAQState.vi"("error in (no error)"=w820, "status"=Status--enum."started", "Instrument.DAQ"=w823) -> ("error out"=w821:errorcluster, "Instrument.DAQ out"=w824:refnum<class "Instrument.DAQ.lvclass">)  [unwired: 7 in]
                n421 = call "DAQ.getSweepWaveforms.vi"("error in (no error)"=w821, "SweepWFMs"=w822, "Instrument.DAQ"=w824) -> ("error out"=w825:errorcluster)  [unwired: 7 in, 1 out]
              }
            }
            n422 = Bundle By Name(cluster=w813, "SweepWaveforms"=w794) -> (w814:T19)
            n423 = flat-sequence {
              tunnel: [w827] -> w802
              tunnel: w797 -> [w826]
              tunnel: [w826] -> w803
              frame #0 {
                n424 = call <vilib>:"High Resolution Relative Seconds.vi"() -> ("relative seconds"=w827:dbl)
              }
            }
            n425 = Subtract(x=w802, y=w799) -> (x-y=→"Sweep Chart":dbl)
            n426 = call <vilib>:"Add State(s) to Queue__jki_lib_state_machine.vi"("State(s) in (\"\")"=w817) -> ("States Out"=w816:string)  [unwired: 14 in]
          }
          frame "Data: Save Intermediate Sweep Data" {
            n427 = call <userlib>:"Periodic Trigger__ogtk.vi"("time (ms)"=u32 1000) -> ()  [unwired: 12 in, 3 out]
            n428 = case shown="True" FALSE {
              tunnel: [w839 w845] -> w835
              tunnel: w834 -> [w839 w844]
              tunnel: [w840 w842] -> w833
              tunnel: w832 -> [w840 w841]
              frame False {
              }
              frame True {
                # "periodically publish waveform and clear buffer:\n- save sooner and more often\n- enable longer sweeps\n#todo\nchange to or add buffer for lossless logging"
                n429 = Unbundle By Name(w841) -> ("SMO"=w847:refnum<class "Instrument.DAQ.lvclass">, "SweepWaveforms"=w846:T11)
                n430 = call "DAQ.getSweepWaveforms.vi"("error in (no error)"=w844, "SweepWFMs"=w846, "Instrument.DAQ"=w847) -> ("error out"=w845:errorcluster)  [unwired: 7 in, 1 out]
                n431 = Bundle By Name(cluster=w841, "SweepWaveforms"=T11 {"AO"=[], "AI"=[], "X"=[], "Y"=[]}) -> (w842:T19)
              }
            }
            n432 = call <vilib>:"Add State(s) to Queue__jki_lib_state_machine.vi"("State(s) in (\"\")"=w838) -> ("States Out"=w837:string)  [unwired: 14 in]
          }
          frame "Data: Cleanup" {
            # "Cleanup any data and references, here.\n(this is called automatically, by the Macro: Exit)"
            n433 = Unbundle By Name(w848) -> ("Core.Current VI Reference"=w852:refnum<vi>)
            n434 = Close Reference(reference=w852, error in (no error)=w851) -> (error out=w850:errorcluster)
            n435 = call <vilib>:"Add State(s) to Queue__jki_lib_state_machine.vi"("State(s) in (\"\")"=w854) -> ("States Out"=w853:string)  [unwired: 14 in]
          }
          frame "---------- UI ----------" {
            # "Do not put any code in this frame.\n(It is a separator no-op. You can make a copy of this frame to create a new UI frame)"
            n436 = call <vilib>:"Add State(s) to Queue__jki_lib_state_machine.vi"("State(s) in (\"\")"=w859) -> ("States Out"=w858:string)  [unwired: 14 in]
          }
          frame "UI: Initialize" {
            # "Initialize the User Interface, here.\n(this is called automatically, by the Macro: Init)"
            n437 = call <userlib>:"Fit VI window to Largest Dec__ogtk.vi"("error in (no error)"=w862, "border spacing (2 px)"=0) -> ("error out"=w863:errorcluster)  [unwired: 4 in, 1 out]
            n438 = local write "Tab Control"(enum32{"Default", "Advanced"}."Default" ("Tab Control")) -> ()
            n439 = local write "Method"("" ("String")) -> ()
            n440 = call <vilib>:"Add State(s) to Queue__jki_lib_state_machine.vi"("State(s) in (\"\")"=w868) -> ("States Out"=w867:string)  [unwired: 14 in]
          }
          frame "UI: Wait" {
            # "UI: Wait.\n(use: \"UI: Wait >> time\" (in ms))"
            n441 = Scan From String(format string="%d", input string=w869, default 1=u32 0 ("default value 1")) -> (output 1=w877:u32)  [unwired: 2 in, 3 out]
            n442 = feedback #1(TRUE ("Triggered")) -> (w874:bool)
            n443 = call <userlib>:"Periodic Trigger__ogtk.vi"("time (ms)"=w877, "reset"=w874) -> ("Triggered"=w875:bool)  [unwired: 11 in, 2 out]
            n444 = feedback-in #1(w875) -> ()
            n445 = call <vilib>:"Build State String with Arguments__JKI_lib_State_Machine.vi"("Arguments (\"\")"=w869, "State"=w873) -> ("State with Arguments"=w872:string)  [unwired: 4 in]
            n446 = Select(t="", s=w875, f=w872) -> (s? t:f=w870:string)
            n447 = call <vilib>:"Add State(s) to Queue__jki_lib_state_machine.vi"("State(s) in Front (\"\")"=w870, "State(s) in (\"\")"=w884) -> ("States Out"=w883:string)  [unwired: 13 in]
          }
          frame "UI: Cursor Set" {
            # "Argument"
            # "Initialize the User Interface, here.\n(this is called automatically, by the Macro: Init)"
            n448 = disable-structure shown="Default" {
              disable-tunnel: w887 -> [w892 w895]
              disable-tunnel: [w892 w894] -> w886
              disable-tunnel: w885 -> [_ w893]
              frame condition #0 {
              }
              frame condition #1 (active) {
                n449 = case shown="\"Idle\", Default" w893 {
                  tunnel: w895 -> [w897 w899]
                  tunnel: [w896 w898] -> w894
                  frame "Idle", Default {
                    n450 = call <vilib>:"Unset Busy.vi"("error in (no error)"=w897) -> ("error out"=w896:errorcluster)  [unwired: 10 in]
                  }
                  frame "Busy" {
                    n451 = call <vilib>:"Set Busy.vi"("error in (no error)"=w899) -> ("error out"=w898:errorcluster)  [unwired: 9 in, 1 out]
                  }
                }
              }
            }
            n452 = call <vilib>:"Add State(s) to Queue__jki_lib_state_machine.vi"("State(s) in (\"\")"=w891) -> ("States Out"=w890:string)  [unwired: 14 in]
          }
          frame "UI: Front Panel State" {
            # "Argument"
            # "Set Front Panel Open or Closed\n(Usage: \"UI: Front Panel State >> Open|Close\")"
            n453 = Unbundle By Name(w903) -> ("Core.Current VI Reference"=w902:refnum<vi>)
            n454 = disable-structure shown="Default" {
              disable-tunnel: w905 -> [w911 w934]
              disable-tunnel: [w910 w934] -> w904
              disable-tunnel: w902 -> [w909 _]
              disable-tunnel: w901 -> [w908 _]
              frame condition #0 (active) {
                n455 = case shown="\"Close\"" w908 {
                  tunnel: w911 -> [w915 w928]
                  tunnel: [w917 w929] -> w910
                  tunnel: w909 -> [w916 w926]
                  frame "Open", Default {
                    n456 = property class="VI"(reference=w916, error in=w915) -> (reference out=w913:refnum<vi>, error out=w914:errorcluster, "FP.State"=w912:T12)
                    n457 = case shown="\"Closed\"" w912 {
                      tunnel: [w920 w923] -> w917
                      tunnel: w914 -> [w919 w923]
                      tunnel: w913 -> [w918 _]
                      frame "Closed" {
                        n458 = invoke class="VI" method="FP.Open"(reference=w918, error in=w919, "Activate"=TRUE, "State"=T12."Standard") -> (error out=w920:errorcluster)  [unwired: 1 in, 4 out]
                      }
                      frame Default {
                      }
                    }
                  }
                  frame "Close" {
                    n459 = property class="VI"(reference=w926, error in=w928) -> (reference out=w925:refnum<vi>, error out=w927:errorcluster, "FP.State"=w924:T12)
                    n460 = case shown="Default" w924 {
                      tunnel: [w930 w933] -> w929
                      tunnel: w927 -> [w930 w932]
                      tunnel: w925 -> [_ w931]
                      frame "Invalid", "Closed" {
                      }
                      frame Default {
                        n461 = invoke class="VI" method="FP.Close"(reference=w931, error in=w932) -> (error out=w933:errorcluster)  [unwired: 1 in, 2 out]
                      }
                    }
                  }
                }
              }
              frame condition #1 {
              }
            }
            n462 = call <vilib>:"Add State(s) to Queue__jki_lib_state_machine.vi"("State(s) in (\"\")"=w907) -> ("States Out"=w906:string)  [unwired: 14 in]
          }
          frame "---------- Macro ----------" {
            # "Do not put any code in this frame.\n(It is a separator no-op. You can make a copy of this frame to create a new Macro frame)"
            n463 = call <vilib>:"Add State(s) to Queue__jki_lib_state_machine.vi"("State(s) in (\"\")"=w939) -> ("States Out"=w938:string)  [unwired: 14 in]
          }
          frame "Macro: Initialize" {
            w942 = "UI: Initialize\nUI: Front Panel State >> Close\nMacro: Debug"  # UI: Initialize UI: Front Panel State >> Close Macro: Debug
            # "Initialization Macro\n(This is called once, when the VI starts)"
            n464 = call <vilib>:"Add State(s) to Queue__jki_lib_state_machine.vi"("State(s) in Front (\"\")"="Data: Initialize\nInitialize Core Data\nEvents: Register", "State(s) in (\"\")"="Process: Sync", "State(s) at Back (\"\")"=w942) -> ("States Out"=w941:string)  [unwired: 12 in]
            n465 = call <vilib>:"Add State(s) to Queue__jki_lib_state_machine.vi"("State(s) in Front (\"\")"=w941, "State(s) in (\"\")"=w948) -> ("States Out"=w947:string)  [unwired: 13 in]
          }
          frame "Macro: Debug" {
            # "exe?"
            # "If pane is an EXE, then close it when we exit"
            # "Macro: Debug\n(get debug behavior, determine UI and determine shutdown behavior)"
            n466 = Unbundle By Name(w951) -> ("Core.Close Panel on Exit?"=w955:bool, "SMO"=w960:refnum<class "Instrument.DAQ.lvclass">)
            n467 = property class="App"() -> ("App.Kind"=w958:T10)  [unwired: 2 in, 2 out]
            n468 = Equal?(x=w958, y=T10."Run Time System" ("Application:Kind")) -> (x = y?=w954:bool)
            n469 = call <userlib>:"Get Debug Mode.vi"("error in (no error)"=w949, "SMO"=w960) -> ("error out"=w950:errorcluster, "Behavior"=w959:T73)  [unwired: 7 in, 1 out]
            n470 = case shown="\"Normal\", Default" w959 {
              tunnel: [w964 w966] -> w956
              tunnel: w955 -> [w964 _]
              tunnel: w954 -> [_ w968]
              tunnel: [_ "UI: Front Panel State >> Open\nUI: Wait >> 1000"] -> w952
              frame "Normal", Default {
                # "respect core.close"
              }
              frame "Debug" {
                # "keep panel open\nunless exe"
                n471 = Or(x=w968, y=FALSE) -> (x .or. y?=w966:bool)
              }
            }
            n472 = Bundle By Name(cluster=w951, "Core.Close Panel on Exit?"=w956) -> (w953:T19)
            n473 = call <vilib>:"Add State(s) to Queue__jki_lib_state_machine.vi"("State(s) in Front (\"\")"=w952, "State(s) in (\"\")"=w963) -> ("States Out"=w962:string)  [unwired: 13 in]
          }
          frame "Macro: Post Error Handling" {
            # "Clear Last Error?"
            # "Handle any errors here.\nYou can also output any states to clean-up after errors occur"
            n474 = Unbundle By Name(w971) -> ("Core.Last Error.error"=w970:errorcluster, "Core.Last Error.remaining states"=w974:string, "Core.Shutdown?"=w975:bool, "SMO"=w969:refnum<class "Instrument.DAQ.lvclass">)
            n475 = Unbundle By Name(w971) -> ("Core.Last Error.error"=w978:errorcluster)
            n476 = case shown="True" FALSE {
              tunnel: w978 -> [w999 _]
              tunnel: [w999 _] -> w977
              frame False {
              }
              frame True {
              }
            }
            n477 = case shown="False" w975 {
              tunnel: w974 -> [_ w998]
              tunnel: [w984 w997] -> w973
              tunnel: w970 -> [w985 _]
              tunnel: w969 -> [w983 _]
              frame False {
                # "These are the remaining states (at the moment the error occured). States can be altered according to business logic."
                # "NOT SHUTTING DOWN"
                n478 = while {
                  tunnel: w985 -> [w991]
                  shift-right: [w991] -> _
                  shift-left: _ -> [w995]
                  tunnel: [w986] -> w984
                  tunnel: w983 -> [w990]
                  stop <- TRUE stop-if-true
                  n479 = Equal?(x=w995, y=w991) -> (x = y?=w992:bool)
                  n480 = call "DAQ.ErrorHandler.vi"("error in (no error)"=w991, "Lockin.DAQ in"=w990) -> ("DAQmx Error?"=w989:bool)  [unwired: 6 in, 3 out]
                  n481 = Select(t="DAQ: STOP", s=w992, f="Idle" ("States Out")) -> (s? t:f=w987:string)
                  n482 = Select(t=w987, s=w989, f="") -> (s? t:f=w986:string)
                }
              }
              frame True {
                # "Developer can decide to alter the states but should be aware that during the shutdown process, there are certain states that must be run for the SMO to properly shut itself (and this process) down. As such, one can add states to perform additional clean-ups, but should append the remaining state to be executed."
                # "SHUTTING DOWN"
                n483 = call <vilib>:"Add State(s) to Queue__jki_lib_state_machine.vi"("State(s) in (\"\")"=w998) -> ("States Out"=w997:string)  [unwired: 14 in]
              }
            }
            n484 = Bundle By Name(cluster=w971, "Core.Last Error.error"=w977) -> (w972:T19)
            n485 = call <vilib>:"Add State(s) to Queue__jki_lib_state_machine.vi"("State(s) in Front (\"\")"=w973, "State(s) in (\"\")"=w982) -> ("States Out"=w981:string)  [unwired: 13 in]
          }
          frame "Macro: Exit" {
            # "Exit Macro\n(This is called once, when the VI exits)"
            n486 = Unbundle By Name(w1000) -> ("Core.Close Panel on Exit?"=w1013:bool)
            n487 = Bundle By Name(cluster=w1000, "Core.Shutdown?"=TRUE) -> (w1001:T19)
            n488 = Select(t="UI: Front Panel State >> Close", s=w1013, f="") -> (s? t:f=w1010:string)
            n489 = call <vilib>:"Add State(s) to Queue__jki_lib_state_machine.vi"("State(s) in Front (\"\")"="Data: Cleanup\nEvents: Unregister", "State(s) in (\"\")"="Process: Sync", "State(s) at Back (\"\")"="Exit") -> ("States Out"=w1007:string)  [unwired: 12 in]
            n490 = call <vilib>:"Add State(s) to Queue__jki_lib_state_machine.vi"("State(s) in Front (\"\")"="Macro: Stop DAQmx", "State(s) in (\"\")"=w1010, "State(s) at Back (\"\")"=w1007) -> ("States Out"=w1005:string)  [unwired: 12 in]
            n491 = call <vilib>:"Add State(s) to Queue__jki_lib_state_machine.vi"("State(s) in Front (\"\")"=w1005, "State(s) in (\"\")"=w1016) -> ("States Out"=w1015:string)  [unwired: 13 in]
          }
          frame "Macro: Start DAQmx" {
            # "Macro: Start.\n(checks the status of DAQmx process)"
            n492 = Unbundle By Name(w1018) -> ("DAQmx Status"=w1017:T2)
            n493 = case shown="\"creating\"" w1017 {
              tunnel: ["DAQ: START" ("State(s) in Front (\"\")") "" ("State(s) in Front (\"\")") "" ("State(s) in Front (\"\")") "idle\nMacro: Start DAQmx" ("State(s) in Front (\"\")") "DAQ: START" ("State(s) in Front (\"\")") "" ("State(s) in Front (\"\")") "" ("State(s) in Front (\"\")") "idle\nMacro: Start DAQmx" ("State(s) in Front (\"\")") "idle\nMacro: Start DAQmx" ("State(s) in Front (\"\")") "idle\nMacro: Start DAQmx" ("State(s) in Front (\"\")")] -> w1019
              frame "idle", Default {
              }
              frame "calibrating" {
              }
              frame "configuring" {
              }
              frame "creating" {
              }
              frame "created" {
              }
              frame "starting" {
              }
              frame "started" {
              }
              frame "stopping" {
              }
              frame "stopped" {
              }
              frame "clearing" {
              }
            }
            n494 = call <vilib>:"Add State(s) to Queue__jki_lib_state_machine.vi"("State(s) in Front (\"\")"=w1019, "State(s) in (\"\")"=w1023) -> ("States Out"=w1022:string)  [unwired: 13 in]
          }
          frame "Macro: Stop DAQmx" {
            # "Macro: Stop.\n(checks the status of DAQmx process)"
            n495 = Unbundle By Name(w1034) -> ("DAQmx Status"=w1036:T2)
            n496 = case shown="\"stopping\"" w1036 {
              tunnel: ["" ("State(s) in Front (\"\")") "" ("State(s) in Front (\"\")") "" ("State(s) in Front (\"\")") "idle\nMacro: Stop DAQmx" ("State(s) in Front (\"\")") "DAQ: STOP" ("State(s) in Front (\"\")") "idle\nMacro: Stop DAQmx" ("State(s) in Front (\"\")") "DAQ: STOP" ("State(s) in Front (\"\")") "" ("State(s) in Front (\"\")") "" ("State(s) in Front (\"\")") "" ("State(s) in Front (\"\")")] -> w1035
              frame "idle", Default {
              }
              frame "calibrating" {
              }
              frame "configuring" {
              }
              frame "creating" {
              }
              frame "created" {
              }
              frame "starting" {
              }
              frame "started" {
              }
              frame "stopping" {
              }
              frame "stopped" {
              }
              frame "clearing" {
              }
            }
            n497 = call <vilib>:"Add State(s) to Queue__jki_lib_state_machine.vi"("State(s) in Front (\"\")"=w1035, "State(s) in (\"\")"=w1040) -> ("States Out"=w1037:string)  [unwired: 13 in]
          }
          frame "Macro: DSP" {
            # "Macro: DSP.\n()"
            n498 = Unbundle By Name(w1060) -> ("SMO"=w1059:refnum<class "Instrument.DAQ.lvclass">)
            n499 = Unbundle By Name(w1059) -> ("AO"=w1052:waveform(dbl)[])
            n500 = call "Get Waveform Sweep Status.vi"("error in (no error)"=w1055, "Waveforms in"=w1052) -> ("error out"=w1056:errorcluster, "sweep status"=w1066:T13)  [unwired: 7 in, 1 out]
            n501 = Equal?(x=w1066, y=Generator.Sweep_Status--enum."sweeping" ("sweep status")) -> (x = y?=w1064:bool)
            n502 = call <userlib>:"Boolean Trigger__ogtk.vi"("Boolean Input"=w1064) -> ("Falling Edge"=w1061:bool)  [unwired: 1 in, 1 out]
            n503 = Select(t="Data: Save Sweep Data" ("State(s) at Back (\"\")"), s=w1064, f="") -> (s? t:f=w1058:string)
            n504 = Select(t="Data: Save Sweep Data >> final" ("State(s) at Back (\"\")"), s=w1061, f="") -> (s? t:f=w1057:string)
            n505 = call <vilib>:"Add State(s) to Queue__jki_lib_state_machine.vi"("State(s) in Front (\"\")"="DSP: Simulate\nDSP: Phase\nDSP: Filter\nDSP: Lockin" ("State(s) in Front (\"\")"), "State(s) in (\"\")"=w1058, "State(s) at Back (\"\")"=w1057) -> ("States Out"=w1053:string)  [unwired: 12 in]
            n506 = call <vilib>:"Add State(s) to Queue__jki_lib_state_machine.vi"("State(s) in Front (\"\")"=w1053, "State(s) in (\"\")"=w1070) -> ("States Out"=w1069:string)  [unwired: 13 in]
          }
          frame "---------- Process ----------" {
            # "Template Separator\n(You can make a copy of, or modify, this frame)"
            n507 = call <vilib>:"Add State(s) to Queue__jki_lib_state_machine.vi"("State(s) in (\"\")"=w1075) -> ("States Out"=w1074:string)  [unwired: 14 in]
          }
          frame "Process: Sync" {
            n508 = Unbundle By Name(w1083) -> ("SMO"=w1079:refnum<class "Instrument.DAQ.lvclass">)
            n509 = call <vilib>:"WaitOnProcessSync.vi"("error in (no error)"=w1078, "SMO"=w1079) -> ("error out"=w1077:errorcluster, "Don't run?"=w1082:bool)  [unwired: 7 in, 1 out]
            n510 = Select(t="Data: Cleanup\nEvents: Unregister\nExit", s=w1082, f="") -> (s? t:f=w1076:string)
            n511 = call <vilib>:"Add State(s) to Queue__jki_lib_state_machine.vi"("State(s) in Front (\"\")"=w1076, "State(s) in (\"\")"=w1086) -> ("States Out"=w1085:string)  [unwired: 13 in]
          }
          frame "---------- Events ----------" {
            # "Template Separator\n(You can make a copy of, or modify, this frame)"
            n512 = call <vilib>:"Add State(s) to Queue__jki_lib_state_machine.vi"("State(s) in (\"\")"=w1091) -> ("States Out"=w1090:string)  [unwired: 14 in]
          }
          frame "Events: Register" {
            n513 = Unbundle By Name(w1109) -> ("SMO"=w1108:refnum<class "Instrument.DAQ.lvclass">)
            n514 = call <vilib>:"GetProtectedEvents.vi"("SMO"=w1108) -> ("error out"=w1106:errorcluster, "SMO Protected Events"=w1105:T74, "SMO out"=w1100:refnum<class "Instrument.DAQ.lvclass">)  [unwired: 8 in]
            n515 = call "DAQ.GetPrivateEvents.vi"("Instrument.DAQ"=w1100) -> ("error out"=w1104:errorcluster, "DAQ Private Events"=w1099:T75, "Instrument.DAQ"=w1102:refnum<class "Instrument.DAQ.lvclass">)  [unwired: 8 in]
            n516 = Unbundle By Name(w1102) -> ("DAQmx"=w1098:refnum<class "DAQmx.lvclass">, "Generator"=w1097:refnum<class "Generator.lvclass">)
            n517 = call "DAQmx.GetPublicEvents.vi"("DAQmx"=w1098) -> ("error out"=w1101:errorcluster, "DAQmx Public Events"=w1092:T76)  [unwired: 8 in, 1 out]
            n518 = call "Generator.GetPublicEvents.vi"("Generator"=w1097) -> ("error out"=w1095:errorcluster, "Generator Public Events"=w1096:T77)  [unwired: 8 in, 1 out]
            n519 = register-events(w1105, w1099, w1092, w1096) -> (reference out=w1103:refnum<event-registration>, error out=w1093:errorcluster)  [unwired: 2 in]
            n520 = Merge Errors(w1094, w1093, w1095, w1101, w1104, w1106) -> (w1107:errorcluster)
            n521 = call <vilib>:"Add State(s) to Queue__jki_lib_state_machine.vi"("State(s) in (\"\")"=w1111) -> ("States Out"=w1110:string)  [unwired: 14 in]
          }
          frame "Events: Unregister" {
            n522 = Unregister For Events(event registration refnum=w1112, error in=w1114) -> (error out=w1113:errorcluster)
            n523 = call <vilib>:"Clear Errors.vi"("error in (no error)"=w1113) -> ()  [unwired: 5 in, 2 out]
            n524 = call <vilib>:"Add State(s) to Queue__jki_lib_state_machine.vi"("State(s) in (\"\")"=w1117) -> ("States Out"=w1116:string)  [unwired: 14 in]
          }
          frame "---------- DAQ ----------" {
            n525 = call <vilib>:"Add State(s) to Queue__jki_lib_state_machine.vi"("State(s) in (\"\")"=w1122) -> ("States Out"=w1121:string)  [unwired: 14 in]
          }
          frame "DAQ: AUTO" {
            n526 = Unbundle By Name(w1126) -> ("SMO"=w1128:refnum<class "Instrument.DAQ.lvclass">)
            n527 = call "DAQ.Auto Configure.vi"("error in (no error)"=w1127, "Instrument.DAQ"=w1128) -> ("error out"=w1123:errorcluster, "Instrument.DAQ out"=w1124:refnum<class "Instrument.DAQ.lvclass">)  [unwired: 8 in]
            n528 = Bundle By Name(cluster=w1126, "SMO"=w1124) -> (w1125:T19)
            n529 = call <vilib>:"Add State(s) to Queue__jki_lib_state_machine.vi"("State(s) in (\"\")"=w1131) -> ("States Out"=w1130:string)  [unwired: 14 in]
          }
          frame "DAQ: START" {
            n530 = Unbundle By Name(w1137) -> ("SMO"=w1135:refnum<class "Instrument.DAQ.lvclass">)
            n531 = call "DAQ.Start.vi"("error in"=w1132, "Instrument.DAQ"=w1135) -> ("error out"=w1133:errorcluster, "Instrument.DAQ out"=w1134:refnum<class "Instrument.DAQ.lvclass">)  [unwired: 8 in]
            n532 = Bundle By Name(cluster=w1137, "SMO"=w1134) -> (w1136:T19)
            n533 = call <vilib>:"Add State(s) to Queue__jki_lib_state_machine.vi"("State(s) in (\"\")"=w1140) -> ("States Out"=w1139:string)  [unwired: 14 in]
          }
          frame "DAQ: CALIBRATE" {
            # "calibrate or get calibration"
            n534 = Unbundle By Name(w1150) -> ("SMO"=w1148:refnum<class "Instrument.DAQ.lvclass">)
            n535 = Scan From String(input string=w1142, default 1=PrivateEvents--DAQ.setCalibration."Check" ("setCalibration")) -> (error out=w1141:errorcluster, output 1=w1143:T14)  [unwired: 3 in, 2 out]
            n536 = call <vilib>:"Clear Errors.vi"("error in (no error)"=w1141) -> ()  [unwired: 5 in, 2 out]
            n537 = case shown="\"Calibrate\"" w1143 {
              tunnel: w1148 -> [w1157 w1161]
              tunnel: [w1156 w1160] -> w1145
              tunnel: w1147 -> [w1154 w1159]
              tunnel: [w1155 w1158] -> w1146
              frame "Check" {
                n538 = call "DAQ.Get Calibration.vi"("error in (no error)"=w1154, "Instrument.DAQ in"=w1157) -> ("error out"=w1155:errorcluster, "Instrument.DAQ out"=w1156:refnum<class "Instrument.DAQ.lvclass">)  [unwired: 8 in]
              }
              frame "Calibrate" {
                n539 = call "DAQ.Calibrate.vi"("error in (no error)"=w1159, "Lockin.DAQ in"=w1161) -> ("error out"=w1158:errorcluster, "Lockin.DAQ out"=w1160:refnum<class "Instrument.DAQ.lvclass">)  [unwired: 8 in]
              }
            }
            n540 = Bundle By Name(cluster=w1150, "SMO"=w1145) -> (w1149:T19)
            n541 = call <vilib>:"Add State(s) to Queue__jki_lib_state_machine.vi"("State(s) in (\"\")"=w1153) -> ("States Out"=w1152:string)  [unwired: 14 in]
          }
          frame "DAQ: STOP" {
            n542 = Unbundle By Name(w1167) -> ("SMO"=w1165:refnum<class "Instrument.DAQ.lvclass">)
            n543 = call "DAQ.Stop.vi"("error in (no error)"=w1163, "Instrument.DAQ in"=w1165) -> ("error out"=w1162:errorcluster, "Instrument.DAQ out"=w1164:refnum<class "Instrument.DAQ.lvclass">)  [unwired: 8 in]
            n544 = Bundle By Name(cluster=w1167, "SMO"=w1164) -> (w1166:T19)
            n545 = call <vilib>:"Add State(s) to Queue__jki_lib_state_machine.vi"("State(s) in (\"\")"=w1170) -> ("States Out"=w1169:string)  [unwired: 14 in]
          }
          frame "---------- DSP ----------" {
            n546 = call <vilib>:"Add State(s) to Queue__jki_lib_state_machine.vi"("State(s) in (\"\")"=w1175) -> ("States Out"=w1174:string)  [unwired: 14 in]
          }
          frame "DSP: Simulate" {
            n547 = Unbundle By Name(w1178) -> ("SMO"=w1182:refnum<class "Instrument.DAQ.lvclass">)
            n548 = call "DAQ.Simulate Noisy AI.vi"("Waveguide Cluster"=T15 {"I+"=0, "I-"=1, "V+"=2, "V-"=3, "Vsg"=4}, "error in (no error)"=w1180, "Instrument.DAQ in"=w1182) -> ("error out"=w1181:errorcluster, "Instrument.DAQ out"=w1177:refnum<class "Instrument.DAQ.lvclass">)  [unwired: 5 in, 2 out]
            n549 = Bundle By Name(cluster=w1178, "SMO"=w1177) -> (w1179:T19)
            n550 = call <vilib>:"Add State(s) to Queue__jki_lib_state_machine.vi"("State(s) in (\"\")"=w1185) -> ("States Out"=w1184:string)  [unwired: 14 in]
          }
          frame "DSP: Phase" {
            # "unused"
            n551 = Unbundle By Name(w1201) -> ("SMO"=w1194:refnum<class "Instrument.DAQ.lvclass">, "Results"=w1193:T18)
            n552 = call "Set REF Phase to Zero.vi"("error in (no error)"=w1198, "Reset Phase"="Reset REF", "Instrument.DAQ"=w1194) -> ("error out"=w1188:errorcluster, "Instrument.DAQ out"=w1190:refnum<class "Instrument.DAQ.lvclass">)  [unwired: 7 in]
            n553 = case shown="True" "Auto Phase" {
              tunnel: w1190 -> [w1207 w1211]
              tunnel: [w1207 w1210] -> w1189
              tunnel: w1188 -> [w1206 w1209]
              tunnel: [w1206 w1208] -> w1187
              frame False {
              }
              frame True {
                n554 = call "PLL.vi"("error in (no error)"=w1209, "Instrument.DAQ in"=w1211) -> ("error out"=w1208:errorcluster, "Instrument.DAQ out"=w1210:refnum<class "Instrument.DAQ.lvclass">)  [unwired: 6 in, 2 out]
              }
            }
            n555 = call "Calibrate Phase.vi"("error in (no error)"=w1187, "Boolean"="Calibrate Phase", "Results"=w1193, "Instrument.DAQ in"=w1189) -> ("error out"=w1196:errorcluster, "Instrument.DAQ out"=w1195:refnum<class "Instrument.DAQ.lvclass">)  [unwired: 6 in]
            n556 = flat-sequence {
              tunnel: w1196 -> [w1213]
              tunnel: [w1213] -> w1192
              frame #0 {
                n557 = local write "Calibrate Phase"(FALSE) -> ()
              }
            }
            n558 = call "Replace AO and REF Ch.vi"("error in (no error)"=w1192, "Instrument.DAQ (NEW)"=w1195, "Instrument.DAQ (OLD)"=w1194) -> ("error out"=w1191:errorcluster, "Instrument.DAQ out"=w1199:refnum<class "Instrument.DAQ.lvclass">)  [unwired: 7 in]
            n559 = Bundle By Name(cluster=w1201, "SMO"=w1199) -> (w1200:T19)
            n560 = call <vilib>:"Add State(s) to Queue__jki_lib_state_machine.vi"("State(s) in (\"\")"=w1205) -> ("States Out"=w1204:string)  [unwired: 14 in]
          }
          frame "DSP: Filter" {
            # "publish waveforms"
            # "does not put filtered waveforms on class wire"
            n561 = Unbundle By Name(w1232) -> ("SMO"=w1230:refnum<class "Instrument.DAQ.lvclass">)
            n562 = call "Subtract DAQ Offset.vi"("error in (no error)"=w1229, "Instrument.DAQ"=w1230) -> ("error out"=w1222:errorcluster, "Instrument.DAQ out"=w1216:refnum<class "Instrument.DAQ.lvclass">)  [unwired: 8 in]
            n563 = Unbundle By Name(w1216) -> ("AO"=w1227:waveform(dbl)[], "AI"=w1215:waveform(dbl)[], "REF_X"=w1225:waveform(dbl)[], "REF_Y"=w1224:waveform(dbl)[], "X"=w1226:waveform(dbl)[], "Y"=w1218:waveform(dbl)[])
            n564 = call "Prefilter.vi"("error in (no error)"=w1222, "Waveforms in"=w1215, "Instrument.DAQ in"=w1216) -> ("error out"=w1220:errorcluster, "Waveforms out"=w1214:waveform(dbl)[], "Instrument.DAQ out"=w1221:refnum<class "Instrument.DAQ.lvclass">)  [unwired: 6 in]
            n565 = Bundle By Name(cluster=T16 {"AO"=[], "AI"=[], "REF_X"=[], "REF_Y"=[], "X"=[], "Y"=[]} ("Waveforms"), "AO"=w1227, "AI"=w1214, "REF_X"=w1225, "REF_Y"=w1224, "X"=w1226, "Y"=w1218) -> (w1223:T16)
            n566 = call "DAQ.getWaveforms.vi"("error in (no error)"=w1220, "Waveforms"=w1223, "Instrument.DAQ"=w1221) -> ("error out"=w1219:errorcluster, "Instrument.DAQ"=w1217:refnum<class "Instrument.DAQ.lvclass">)  [unwired: 7 in]
            n567 = Bundle By Name(cluster=w1232, "SMO"=w1217) -> (w1231:T19)
            n568 = call <vilib>:"Add State(s) to Queue__jki_lib_state_machine.vi"("State(s) in (\"\")"=w1235) -> ("States Out"=w1234:string)  [unwired: 14 in]
          }
          frame "DSP: Lockin" {
            n569 = Unbundle By Name(w1249) -> ("SMO"=w1239:refnum<class "Instrument.DAQ.lvclass">)
            n570 = flat-sequence {
              tunnel: [w1265] -> w1244
              tunnel: w1238 -> [w1264]
              tunnel: [w1264] -> w1247
              frame #0 {
                n571 = call <vilib>:"High Resolution Relative Seconds.vi"() -> ("relative seconds"=w1265:dbl)
              }
            }
            n572 = call "Lockin.Engine.vi"("error in (no error)"=w1247, "Instrument.DAQ"=w1239) -> ("error out"=w1245:errorcluster, "Results (X,Y,R,Theta,Mean)"=w1241:T18, "Instrument.DAQ out"=w1240:refnum<class "Instrument.DAQ.lvclass">, "Continue DSP?"=w1237:bool)  [unwired: 5 in, 1 out]
            n573 = flat-sequence {
              tunnel: [w1263] -> w1246
              tunnel: w1245 -> [w1262]
              tunnel: [w1262] -> w1236
              frame #0 {
                n574 = call <vilib>:"High Resolution Relative Seconds.vi"() -> ("relative seconds"=w1263:dbl)
              }
            }
            n575 = case shown="True" w1237 {
              tunnel: w1249 -> [w1254 w1261]
              tunnel: [w1254 w1260] -> w1248
              tunnel: [w1253 w1258] -> w1243
              tunnel: w1241 -> [_ w1257]
              tunnel: w1240 -> [_ w1256]
              tunnel: w1236 -> [w1253 w1255]
              frame False {
              }
              frame True {
                # "publish Results"
                n576 = call "DAQ.getResults.vi"("error in (no error)"=w1255, "Results"=w1257, "Instrument.DAQ"=w1256) -> ("error out"=w1258:errorcluster, "Instrument.DAQ out"=w1259:refnum<class "Instrument.DAQ.lvclass">)  [unwired: 7 in]
                n577 = Bundle By Name(cluster=w1261, "SMO"=w1259, "Results"=w1257) -> (w1260:T19)
              }
            }
            n578 = Subtract(x=w1246, y=w1244) -> (x-y=→"DSP (s)" →"DSP Chart":dbl)
            n579 = call <vilib>:"Add State(s) to Queue__jki_lib_state_machine.vi"("State(s) in (\"\")"=w1252) -> ("States Out"=w1251:string)  [unwired: 14 in]
          }
          frame "DSP: Route" {
            n580 = Unbundle By Name(w1266) -> ()  [unwired: 1 out]
            n581 = call <vilib>:"Add State(s) to Queue__jki_lib_state_machine.vi"("State(s) in (\"\")"=w1270) -> ("States Out"=w1269:string)  [unwired: 14 in]
          }
          frame "DSP: Measure DAQ Offset" {
            w1284 = FALSE ("measureOffset")
            # "this is only a set method"
            # "multiply by gain to get signal at ADC"
            # "AO/AI divides by gain"
            # "This state happens before any offset is subtracted\n(so no need to subtract any offsets first...)"
            # "reset indicator after measuring"
            n582 = Unbundle By Name(w1287) -> ("SMO"=w1281:refnum<class "Instrument.DAQ.lvclass">)
            n583 = Unbundle By Name(w1281) -> ("AI"=w1271:waveform(dbl)[])
            n584 = call "Multiply Waveform by Input Gain.vi"("error in (no error)"=w1272, "WFM in"=w1271, "Instrument.DAQ"=w1281) -> ("error out"=w1280:errorcluster, "WFM out"=w1278:waveform(dbl)[], "Instrument.DAQ out"=w1282:refnum<class "Instrument.DAQ.lvclass">)  [unwired: 6 in]
            n585 = call-poly <vilib>:"Basic Averaged DC-RMS.vi"("reset"=TRUE, "error in (no error)"=w1280, "signals in"=w1278) -> ("error out"=w1283:errorcluster, "DC values"=w1277:dbl[])  [unwired: 5 in, 2 out]
            n586 = call "Set DAQ Offset.vi"("error in (no error)"=w1283, "Offsets"=w1277, "Instrument.DAQ"=w1282) -> ("error out"=w1274:errorcluster, "Instrument.DAQ out"=w1276:refnum<class "Instrument.DAQ.lvclass">)  [unwired: 7 in]
            n587 = Unbundle By Name(w1276) -> ("Offset_AI"=w1275:T72)
            n588 = call "DAQ.getInputOffset.vi"("error in (no error)"=w1274, "Input Offset"=w1275, "Instrument.DAQ"=w1276) -> ("error out"=w1273:errorcluster, "Instrument.DAQ out"=w1279:refnum<class "Instrument.DAQ.lvclass">)  [unwired: 7 in]
            n589 = Bundle By Name(cluster=w1287, "SMO"=w1279, "Measure Offset"=w1284) -> (w1286:T19)
            n590 = local write "Measure Offset"(w1284) -> ()
            n591 = call <vilib>:"Add State(s) to Queue__jki_lib_state_machine.vi"("State(s) in (\"\")"=w1290) -> ("States Out"=w1289:string)  [unwired: 14 in]
          }
          frame "DSP: Zero DAQ Offset" {
            # "reset indicator after zeroing"
            n592 = Unbundle By Name(w1303) -> ("SMO"=w1301:refnum<class "Instrument.DAQ.lvclass">)
            n593 = Unbundle By Name(w1301) -> ("AI"=w1298:waveform(dbl)[])
            n594 = Array Size(array=w1298) -> (size(s)=w1299:i32)
            n595 = Initialize Array(0.0, w1299) -> (w1291:dbl[])
            n596 = call "Set DAQ Offset.vi"("error in (no error)"=w1300, "Offsets"=w1291, "Instrument.DAQ"=w1301) -> ("error out"=w1295:errorcluster, "Instrument.DAQ out"=w1293:refnum<class "Instrument.DAQ.lvclass">)  [unwired: 7 in]
            n597 = Unbundle By Name(w1293) -> ("Offset_AI"=w1296:T72)
            n598 = call "DAQ.getInputOffset.vi"("error in (no error)"=w1295, "Input Offset"=w1296, "Instrument.DAQ"=w1293) -> ("error out"=w1294:errorcluster, "Instrument.DAQ out"=w1292:refnum<class "Instrument.DAQ.lvclass">)  [unwired: 7 in]
            n599 = local write "Zero Offset"(FALSE ("measureOffset")) -> ()
            n600 = Bundle By Name(cluster=w1303, "SMO"=w1292) -> (w1302:T19)
            n601 = call <vilib>:"Add State(s) to Queue__jki_lib_state_machine.vi"("State(s) in (\"\")"=w1307) -> ("States Out"=w1306:string)  [unwired: 14 in]
          }
          frame "---------- Sweep ----------" {
            n602 = call <vilib>:"Add State(s) to Queue__jki_lib_state_machine.vi"("State(s) in (\"\")"=w1312) -> ("States Out"=w1311:string)  [unwired: 14 in]
          }
          frame "Sweep: Initialize" {
            n603 = Get Date/Time In Seconds() -> (seconds since 1Jan1904=w1315:timestamp)
            n604 = To Double Precision Float(number=w1315) -> (double precision float=→"Sweep Start":dbl)
            n605 = call <vilib>:"Add State(s) to Queue__jki_lib_state_machine.vi"("State(s) in (\"\")"=w1319) -> ("States Out"=w1318:string)  [unwired: 14 in]
          }
          frame "----------  Generator ----------" {
            n606 = call <vilib>:"Add State(s) to Queue__jki_lib_state_machine.vi"("State(s) in (\"\")"=w1324) -> ("States Out"=w1323:string)  [unwired: 14 in]
          }
          frame "Generator: Start" {
            n607 = Unbundle By Name(w1330) -> ("SMO"=w1329:refnum<class "Instrument.DAQ.lvclass">)
            n608 = Unbundle By Name(w1329) -> ("Generator"=w1328:refnum<class "Generator.lvclass">)
            n609 = call "setCommand.vi"("error in (no error)"=w1326, "command"=Generator.Command--enum."start", "Generator in"=w1328) -> ("error out"=w1327:errorcluster)  [unwired: 7 in, 1 out]
            n610 = call <vilib>:"Add State(s) to Queue__jki_lib_state_machine.vi"("State(s) in (\"\")"=w1333) -> ("States Out"=w1332:string)  [unwired: 14 in]
          }
          frame "Generator: Start Sweep" {
            n611 = Unbundle By Name(w1339) -> ("SMO"=w1338:refnum<class "Instrument.DAQ.lvclass">)
            n612 = Unbundle By Name(w1338) -> ("Generator"=w1337:refnum<class "Generator.lvclass">)
            n613 = call "setCommand.vi"("error in (no error)"=w1335, "command"=Generator.Command--enum."start sweep", "Generator in"=w1337) -> ("error out"=w1336:errorcluster)  [unwired: 7 in, 1 out]
            n614 = call <vilib>:"Add State(s) to Queue__jki_lib_state_machine.vi"("State(s) in (\"\")"=w1342) -> ("States Out"=w1341:string)  [unwired: 14 in]
          }
          frame "Generator: Stop" {
            n615 = Unbundle By Name(w1348) -> ("SMO"=w1347:refnum<class "Instrument.DAQ.lvclass">)
            n616 = Unbundle By Name(w1347) -> ("Generator"=w1346:refnum<class "Generator.lvclass">)
            n617 = call "setCommand.vi"("error in (no error)"=w1344, "command"=Generator.Command--enum."stop", "Generator in"=w1346) -> ("error out"=w1345:errorcluster)  [unwired: 7 in, 1 out]
            n618 = call <vilib>:"Add State(s) to Queue__jki_lib_state_machine.vi"("State(s) in (\"\")"=w1351) -> ("States Out"=w1350:string)  [unwired: 14 in]
          }
          frame "Generator: Stop Sweep" {
            n619 = Unbundle By Name(w1357) -> ("SMO"=w1356:refnum<class "Instrument.DAQ.lvclass">)
            n620 = Unbundle By Name(w1356) -> ("Generator"=w1355:refnum<class "Generator.lvclass">)
            n621 = call "setCommand.vi"("error in (no error)"=w1353, "command"=Generator.Command--enum."stop sweep", "Generator in"=w1355) -> ("error out"=w1354:errorcluster)  [unwired: 7 in, 1 out]
            n622 = call <vilib>:"Add State(s) to Queue__jki_lib_state_machine.vi"("State(s) in (\"\")"=w1360) -> ("States Out"=w1359:string)  [unwired: 14 in]
          }
        }
      }
    }
    frame Error {
    }
  }
  n623 = call-parent "Process.vi"("error in"=w5, "SMO"=w4) -> ("error out"=w2:errorcluster, "SMO out"=→"Instrument.DAQ out":refnum<class "Instrument.DAQ.lvclass">)  [unwired: 8 in]
  n624 = Merge Errors(w2, w1) -> (→"error out":errorcluster)
